vi "main.vi"() -> ()   [LabVIEW 2025]
uses:
  System.Windows.Forms
  TraceForwardLabviewAppTrace/Components/UIRefForHostInformation.ctl
  TraceForwardLabviewAppTrace/Components/MachineInterface/items/MachineState.ctl
  FormatData_ctl.ctl
  Mode_ctl.ctl
  TraceForwardLabviewAppTrace/Components/UIRefGlobal.vi
  TraceForwardLabviewAppTrace/Components/Config/items/GlobalConfigParam.vi
  <vilib>/NI/Modbus Library/API/Wrapper/Create Serial Master.vi
  <vilib>/NI/Modbus Library/API/Master/Modbus Master.lvclass
  <vilib>/Utility/config.llb/NI_LVConfig.lvlib
  TraceForwardLabviewAppTrace/Components/MachineInterface/MachineInterface.lvlib
  TraceForwardLabviewAppTrace/Components/HostInterface/HostInterface.lvlib
  TraceForwardLabviewAppTrace/Components/Logging/LogFunction.lvlib
  TraceForwardLabviewAppTrace/Components/Config/ConfigAppTraceFunction.lvlib
  <vilib>/NI/Modbus Library/API/Wrapper/API Main.lvlib
panel:
  out "Job ID":string
  out "QR code":string
  in  "Line":string
  out "标题":string="Nailer打钉功能测试"
  out "Assert Number":string
  out "Connection":bool
  out "HighAlarm":bool
  out "Energy(Wh)":dbl
  out "Power(W)":dbl
  out "Current(A)":dbl
  out "Error message":string
  out "register data":u16[](array[numeric])
  out "isOpen":bool
  out "FirstTime":bool
  out "Title":string
  out "Battery Low Voltage":bool
  out "Battery Voltage":dbl
  in  "Stop":bool
  in  "开始":bool caption="Start"
  out "PLC连接状态":bool caption="PLC Connection State"
  in  "型号":string(combo) caption="Model"
  in  "清零":bool caption="Reset"
  in  "Exit":bool
  in  "设置":bool caption="Setting"
  out "项目":string[][](table)
  out "波形图":waveform(dbl)(graph)
  out "进度条":u8(slide) scale=0.0..10.0
  in  "StatusStrip":refnum<k24>(container)
  # "v1.40"
  # "V"
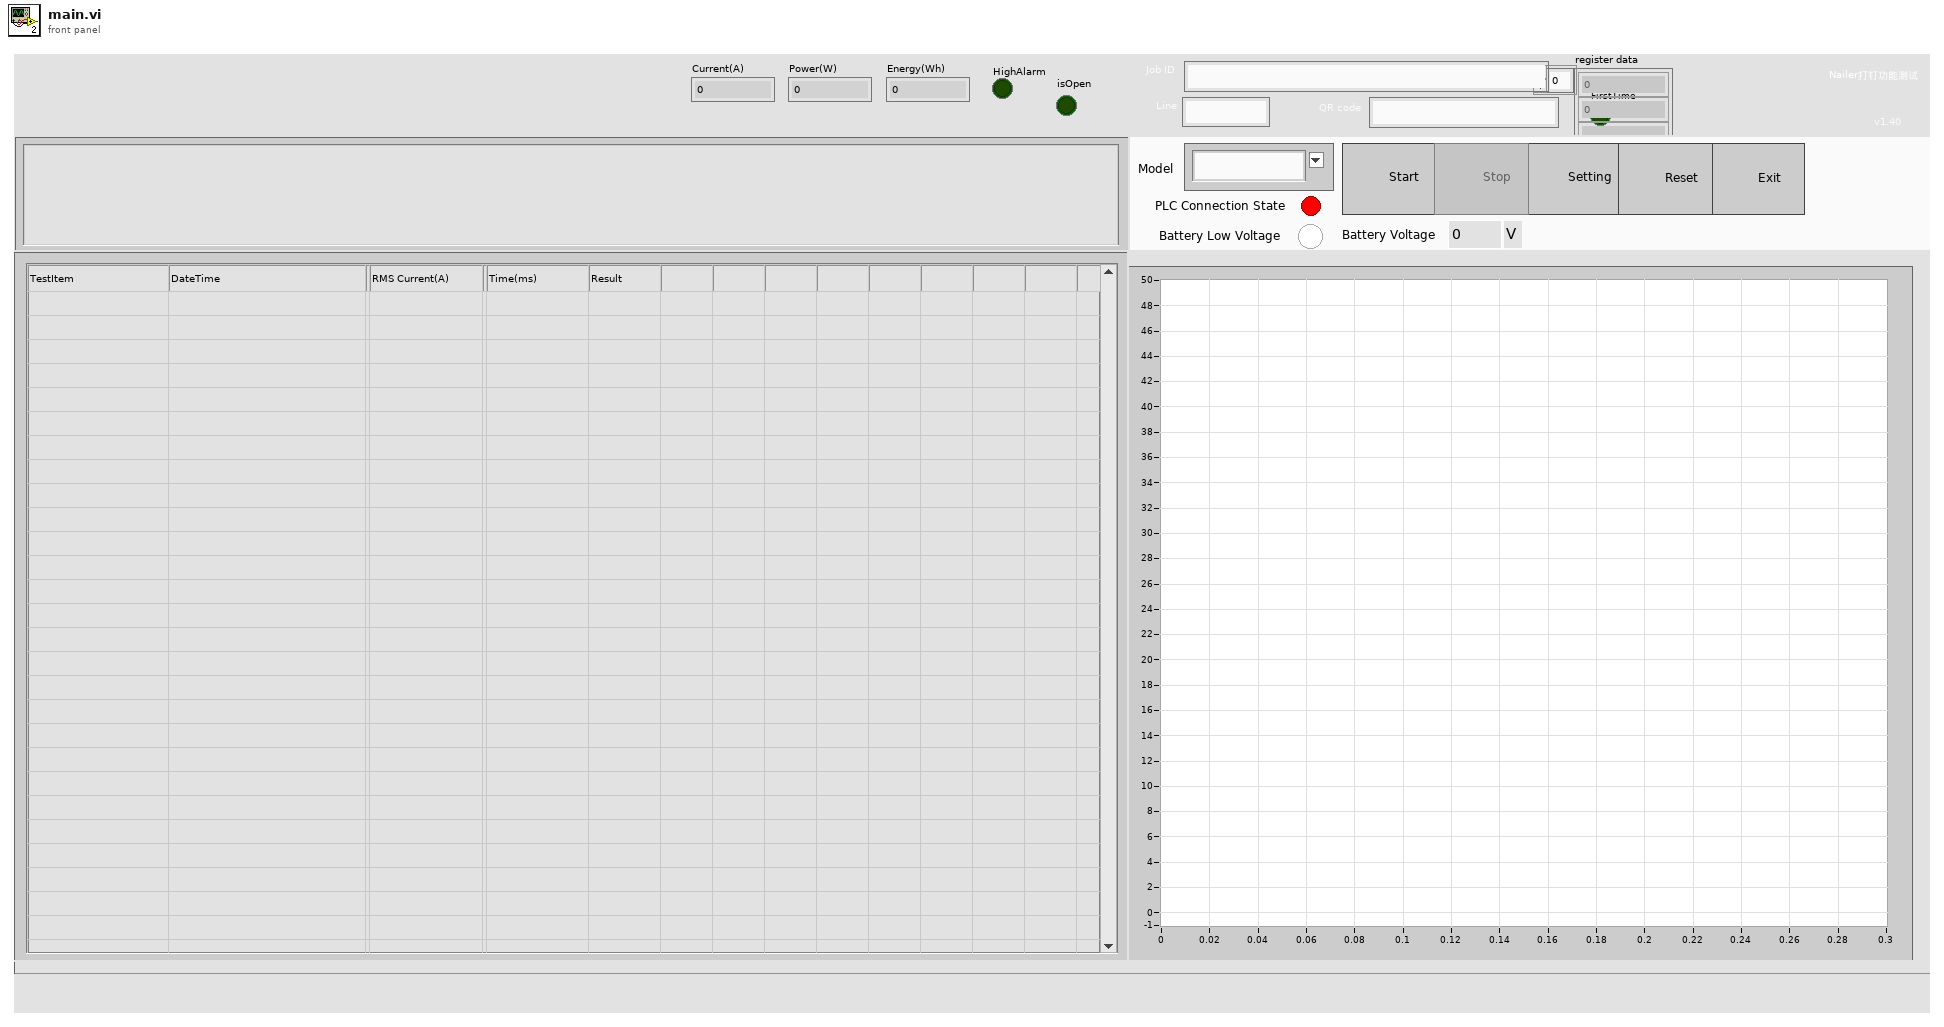
[diagram p1: front panel]
types:
  T1 = typedef "TraceForwardConnection.lvlib/MachineInterface.lvlib/UIRefForHostInformation.ctl" = cluster{"Lost Host Connection":refnum<vi>, "Error message":refnum<vi>, "Job ID":refnum<vi>, "QR":refnum<vi>, "Line id":refnum<vi>, "AssertNumber":refnum<vi>}
  T2 = cluster{"Text Color":u32, "Background Color":u32}
  T3 = enum32{"Invalid", "Standard", "Closed", "Hidden", "Minimized", "Maximized"}
  T4 = typedef "TraceForwardConnection.lvlib/MachineInterface.lvlib/MachineState.ctl" = enum16{"Reset", "Pre-start", "During test", "Data Ready", "OK_NG", "Stop", "WaitMC"}
  T5 = typedef "Mode_ctl.ctl" = enum16{"AddParam", "AddResult", "ReadData", "Clear"}
  T6 = typedef "FormatData_ctl.ctl" = cluster{"Max Current(A)":bool, "Avr Current(A)":bool, "Power":bool, "Time":bool, "Max Current(A) - UpLim":dbl, "Max Current(A) - MinLim":dbl, "Max Current(A) - RealValue":dbl, "Max Current(A) - Result":bool, "Avr Current(A) - UpLim":dbl, "Avr Current(A) - MinLim":dbl, "Avr Current(A) - RealValue":dbl, "Avr Current(A) - Result":bool, "Power- UpLim":dbl, "Power - MinLim":dbl, "Power- RealValue":dbl, "Power - Result":bool, "Time - UpLim":dbl, "Time - MinLim":dbl, "Time-RealValue":dbl, "Time - Result":bool}
  T7 = typedef "NI_LVConfig.lvlib/Config Data RefNum.ctl" = refnum<k1>
  T8 = cluster{"最大电流":bool, "平均电流":bool, "能量":bool, "打钉时间":bool, "单发打钉次数":u32, "连发打钉次数":u32, "触发值":dbl, "平均电流上限":dbl, "平均电流下限":dbl, "最大电流上限":dbl, "最大电流下限":dbl, "能量上限":dbl, "能量下限":dbl, "时间上限":dbl, "时间下限":dbl, "停止值":dbl, "倍数":dbl, "最大补偿":dbl, "平均补偿":dbl, "能量补偿":dbl, "时间补偿":dbl, "检查数":u32, "CurrentType":enum16{"RMS均方根值", "AVG平均值"}}
  T9 = cluster{"Name":string, "Type":string, "DefVal":string}[]
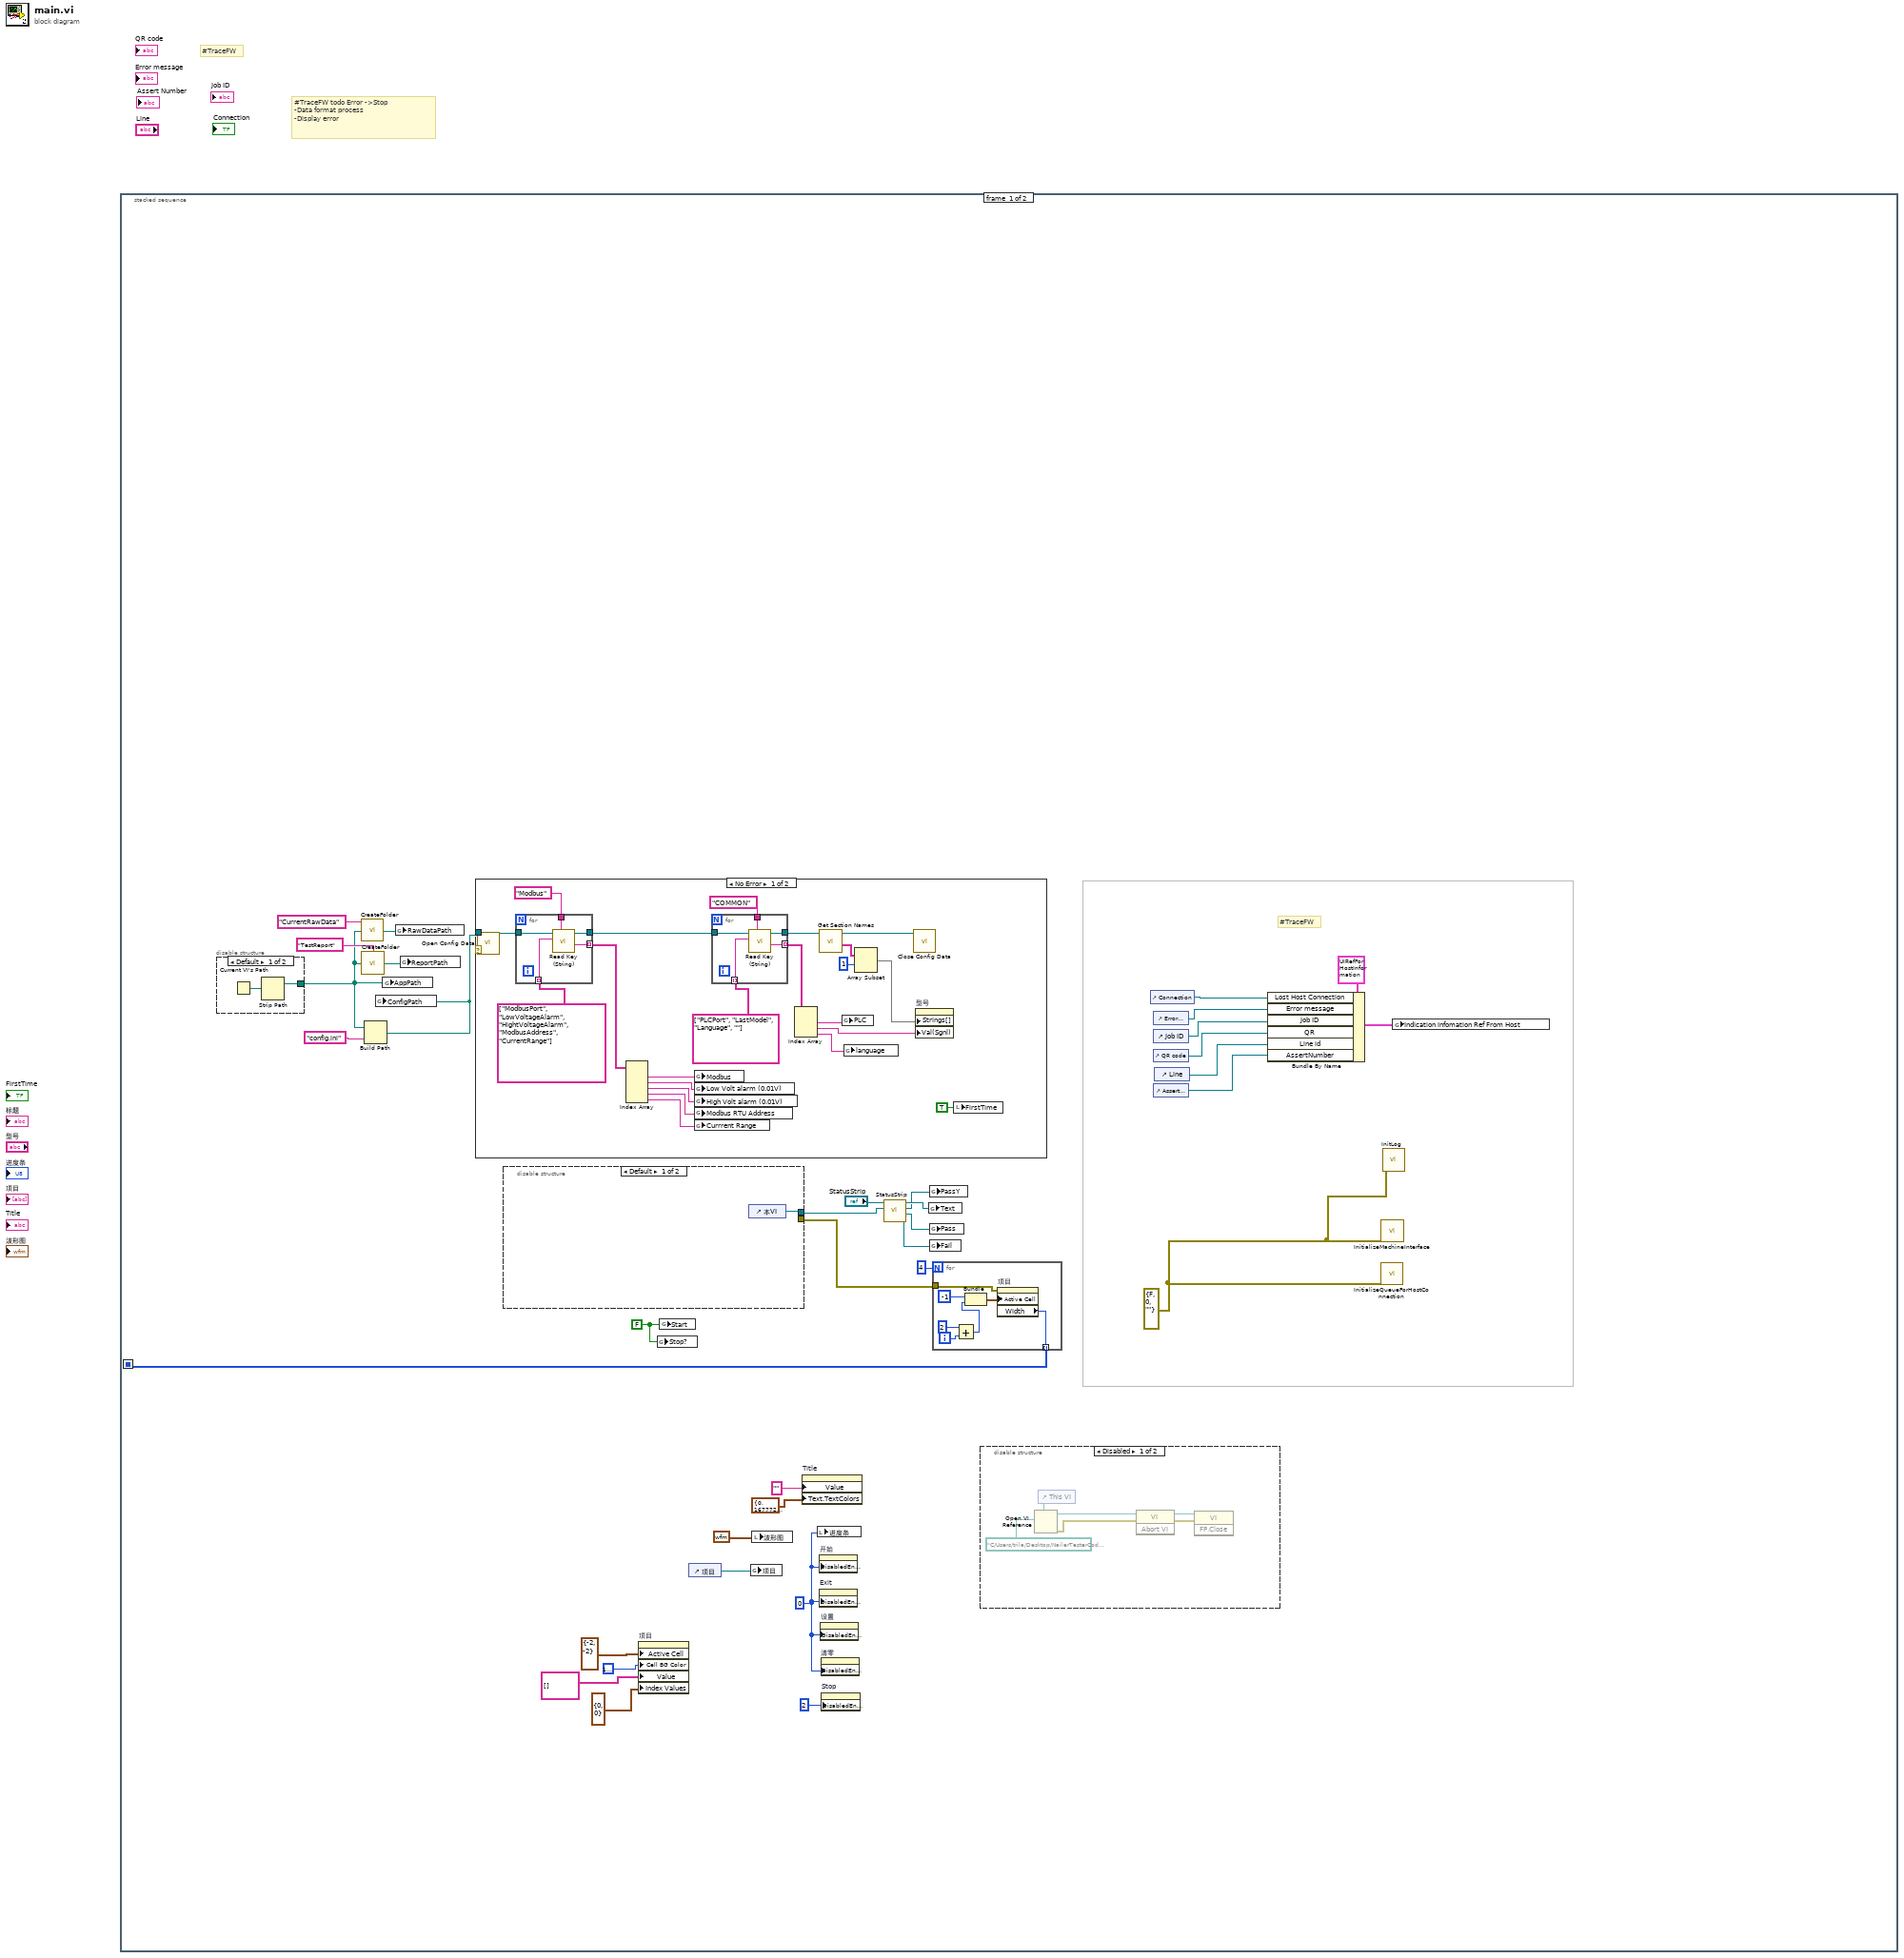
[diagram p0: block diagram]
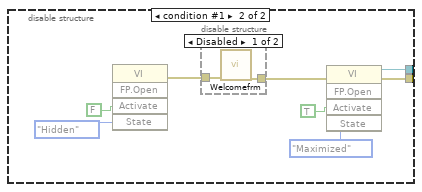
[diagram p3: hidden frame]
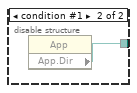
[diagram p5: hidden frame]
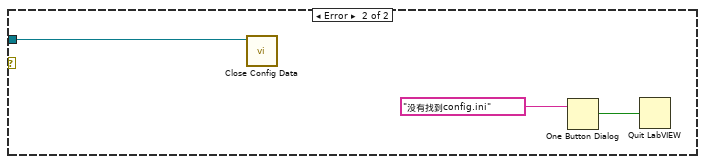
[diagram p6: hidden frame]
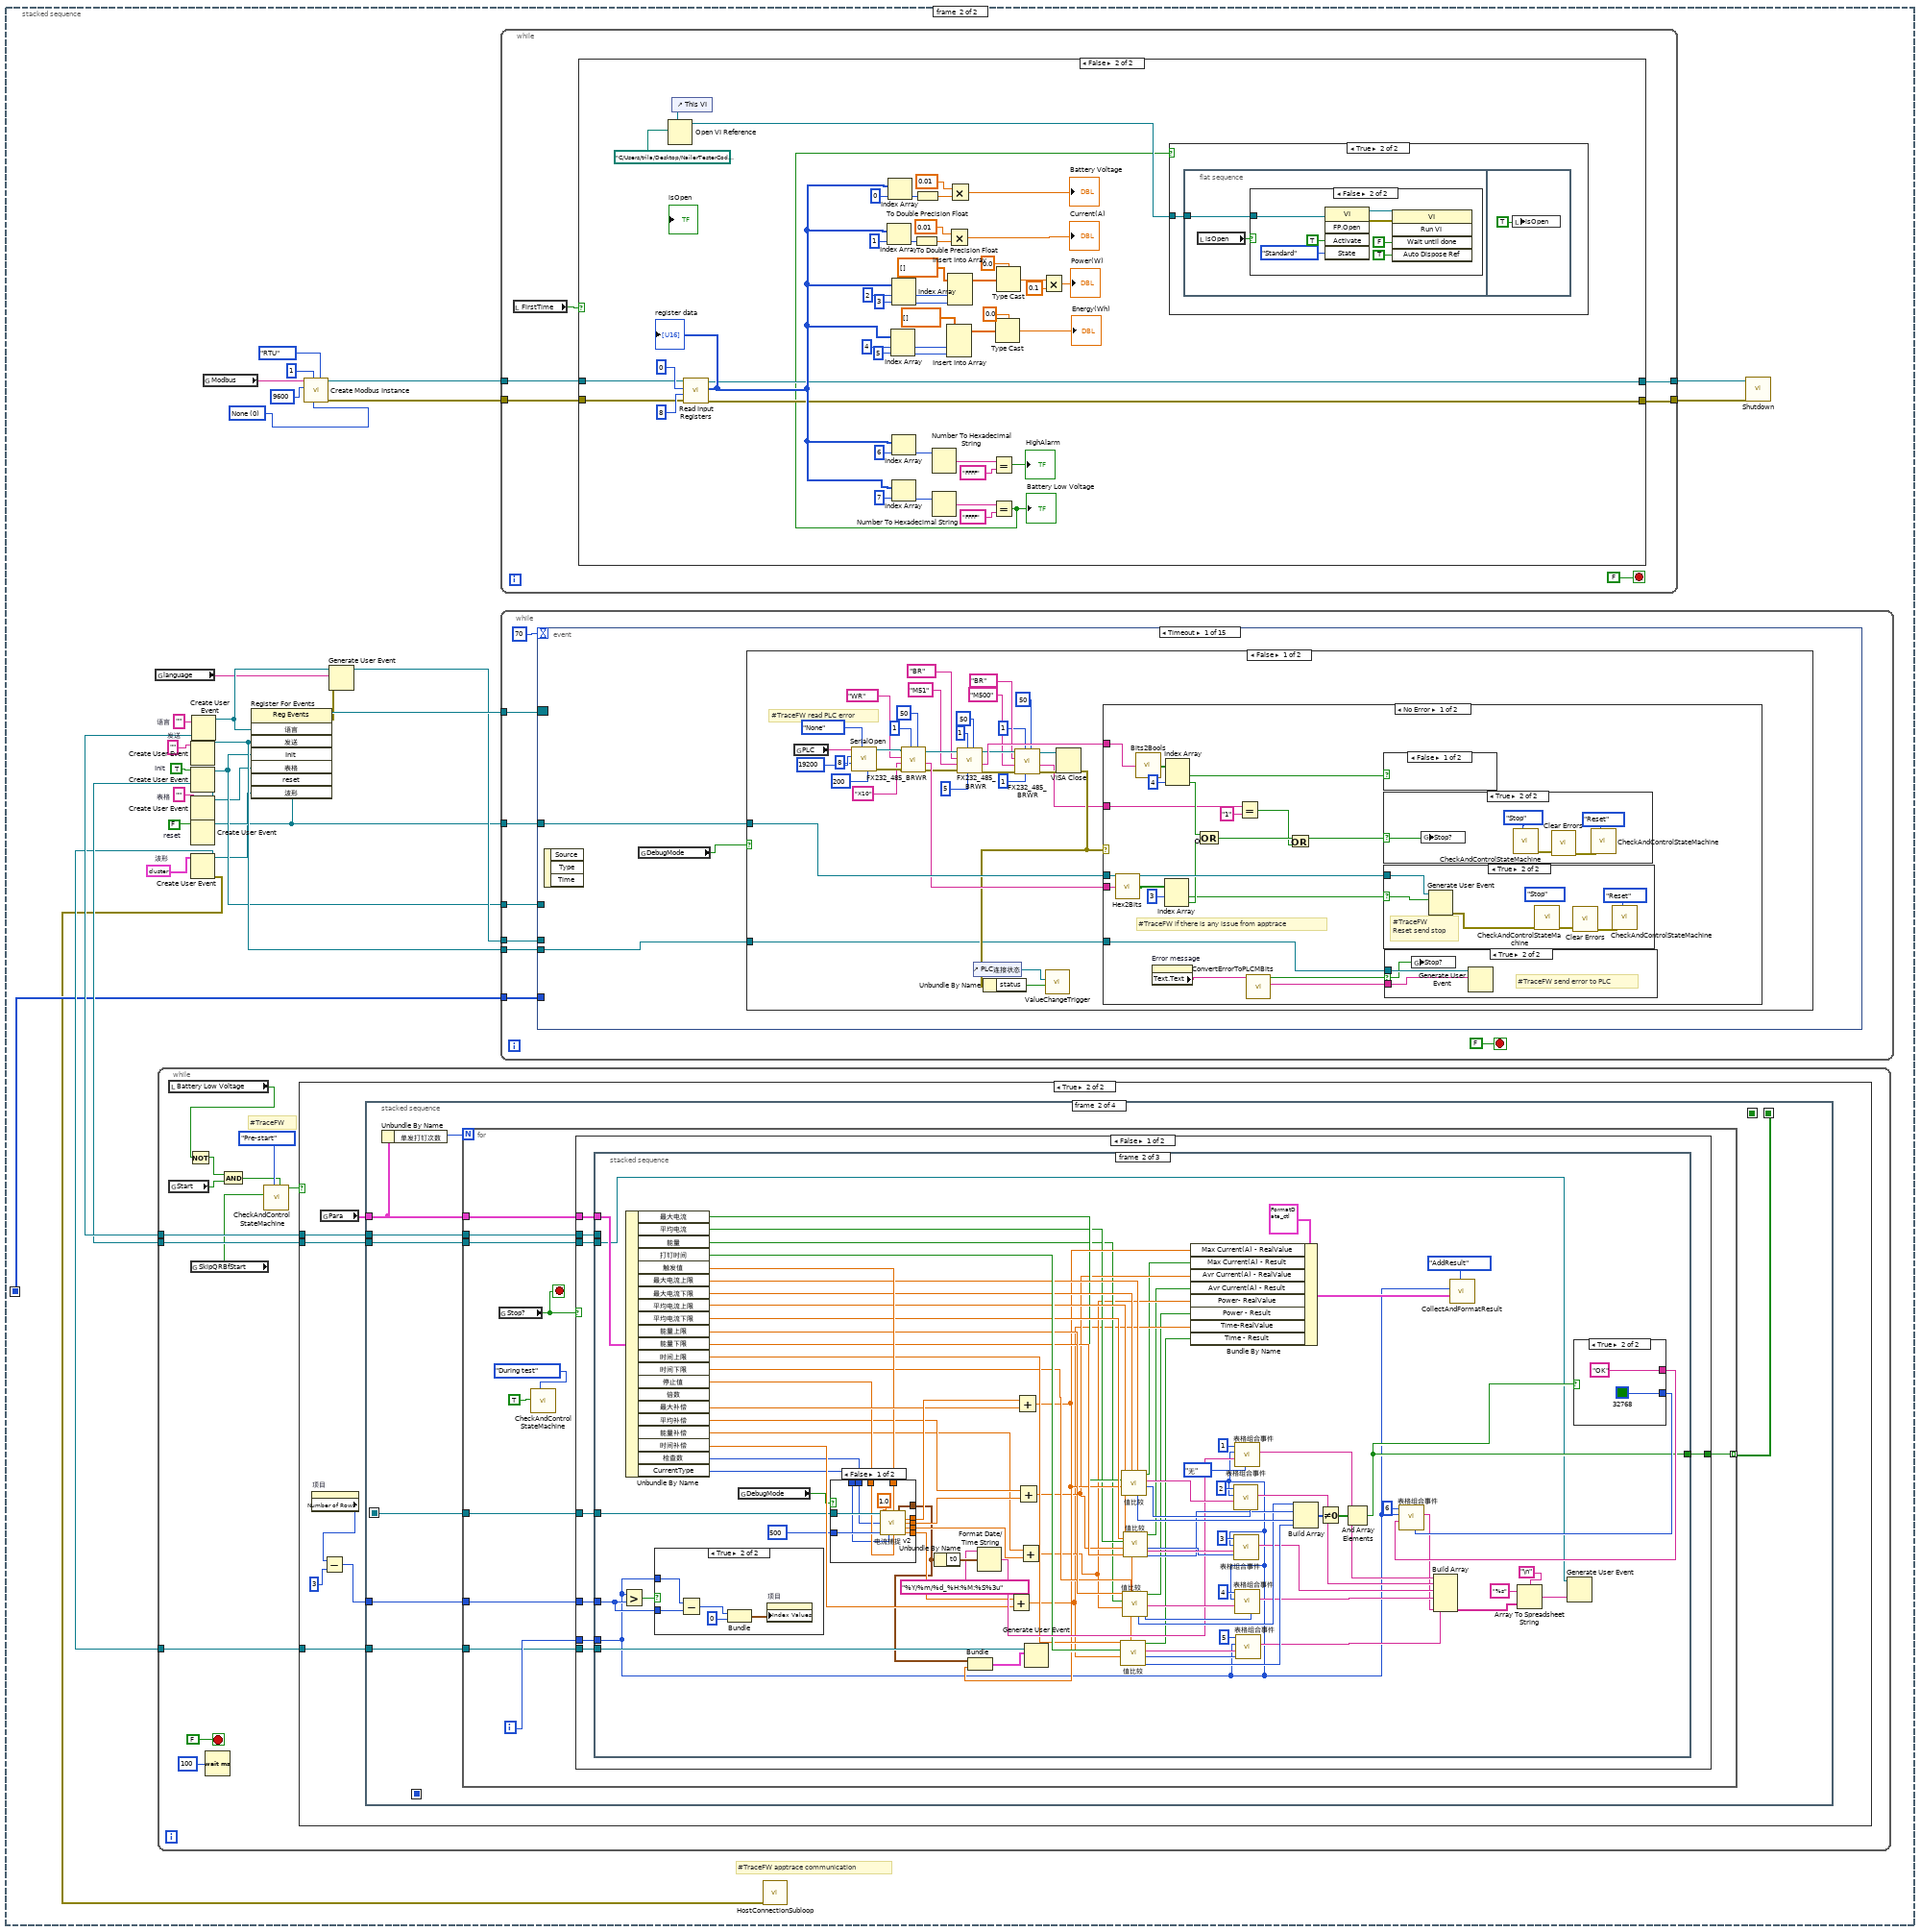
[diagram p7: hidden frame]
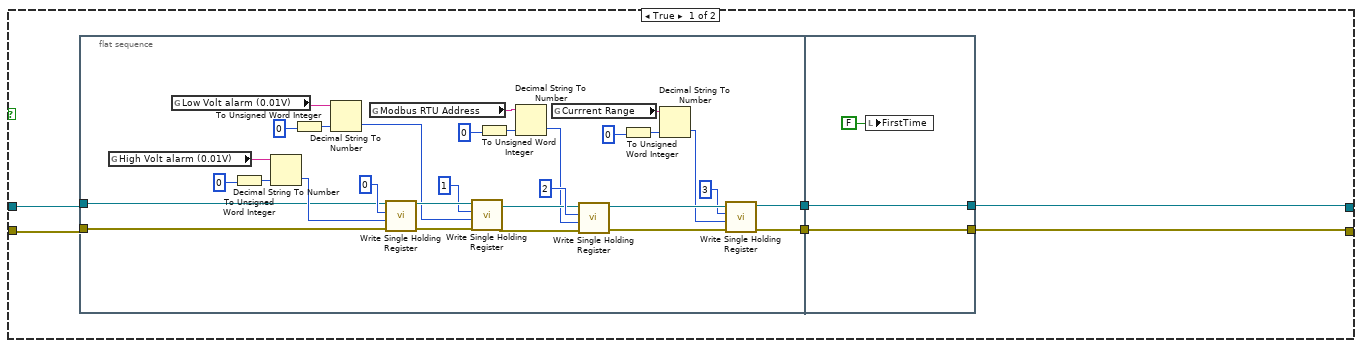
[diagram p8: hidden frame]
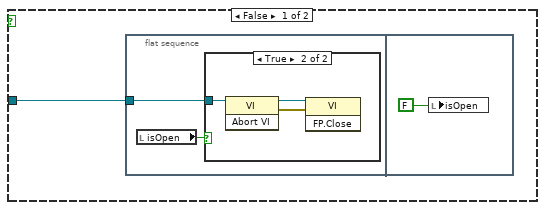
[diagram p9: hidden frame]
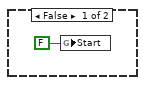
[diagram p12: hidden frame]
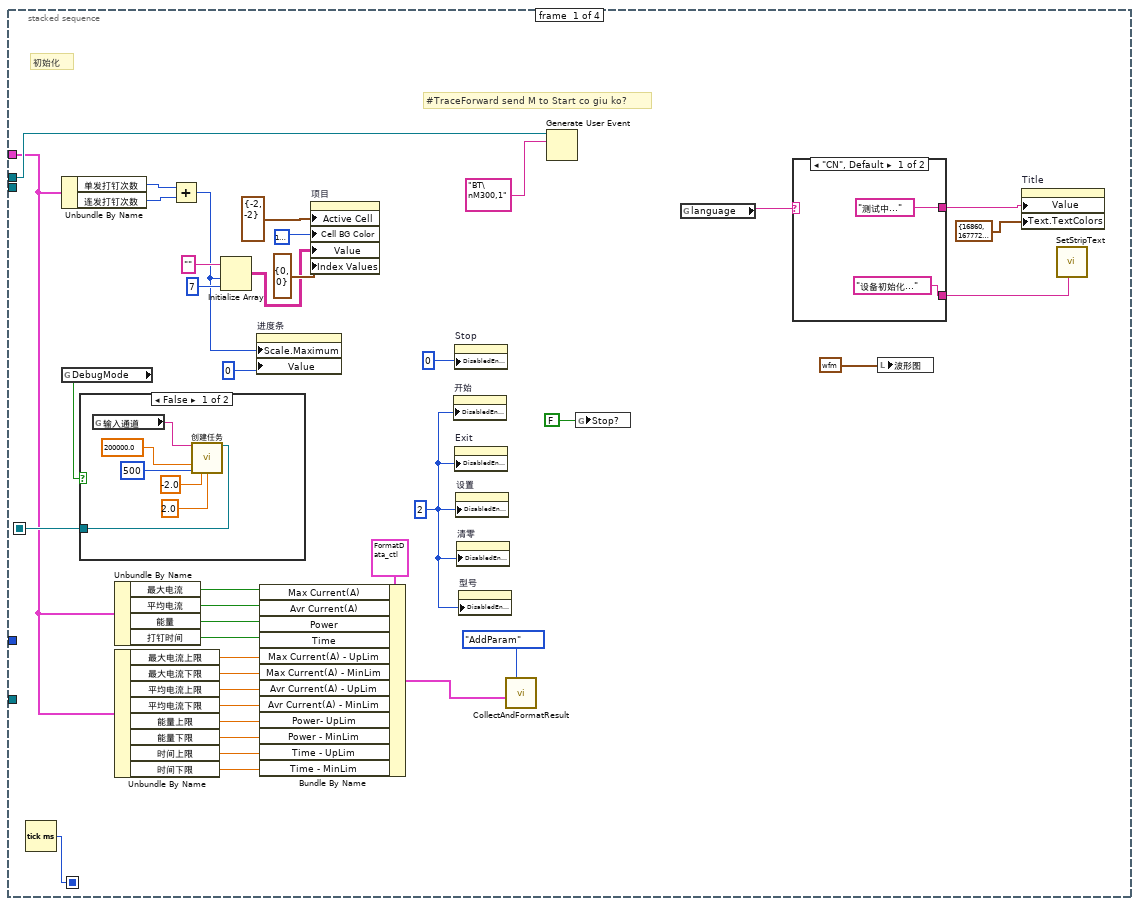
[diagram p13: hidden frame]
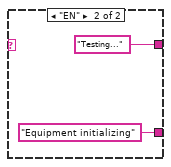
[diagram p15: hidden frame]
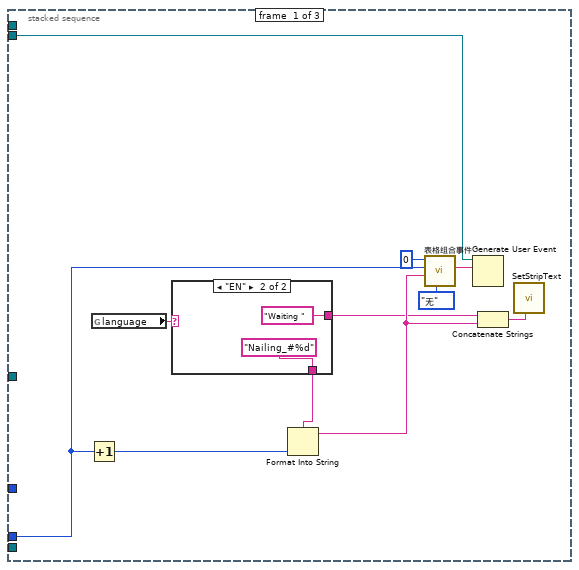
[diagram p16: hidden frame]
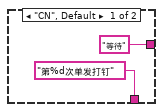
[diagram p17: hidden frame]
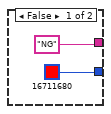
[diagram p20: hidden frame]
diagram:
  # "#TraceFW todo Error ->Stop\n-Data format process\n-Display error"
  # "#TraceFW"
  n1 = stacked-sequence {
    seq-local: [w15 _] -> [_ w113]
    frame #0 {
      w5 = errorcluster {"status"=FALSE, "code"=0, "source"=""} ("error in (no error)")
      w16 = 0
      w18 = FALSE ("InMain")
      # "#TraceFW"
      n2 = disable-structure shown="Default" {
        disable-tunnel: [w64 w66] -> w3
        frame condition #0 (active) {
          n3 = Current VI's Path() -> (path=w65:path)
          n4 = Strip Path(path=w65) -> (stripped path=w64:path)  [unwired: 1 out]
        }
        frame condition #1 {
          n5 = property class="App"() -> ("App.Dir"=w66:path)  [unwired: 2 in, 2 out]
        }
      }
      n6 = call "CreateFolder.vi"("folder name"="CurrentRawData", "Path in"=w3) -> ("path out"=w1:path)  [unwired: 2 in]
      n7 = call "CreateFolder.vi"("folder name"="TestReport" ("名称或相对路径"), "Path in"=w3) -> ("path out"=w22:path)  [unwired: 2 in]
      n8 = Build Path(base path=w3, name or relative path="config.ini" ("名称或相对路径")) -> (appended path=w20:path)
      n9 = global write "global.vi" "ConfigPath"(w20) -> ()
      n10 = global write "global.vi" "AppPath"(w3) -> ()
      n11 = global write "global.vi" "RawDataPath"(w1) -> ()
      n12 = global write "global.vi" "ReportPath"(w22) -> ()
      n13 = call <vilib>:"Open Config Data.vi"("configuration file path"=w20) -> ("error out"=w34:errorcluster, "refnum"=w33:T7)  [unwired: 8 in, 1 out]
      n14 = case shown="No Error" w34 {
        tunnel: w33 -> [w77 w99]
        frame No Error {
          n15 = for {
            tunnel: w77 -> [w93]
            tunnel: "Modbus" ("section") -> [w92]
            tunnel: string[] ["ModbusPort", "LowVoltageAlarm", "HightVoltageAlarm", "ModbusAddress", "CurrentRange"] -> [w91] mode=indexing
            tunnel: [w90] -> w73
            tunnel: [w89] -> w74 mode=indexing
            n16 = call <vilib>:"Read Key (String).vi"("section"=w92, "key"=w91, "refnum"=w93) -> ("value"=w89:string, "refnum out"=w90:T7)  [unwired: 5 in, 2 out]
          }
          n17 = Index Array(array=w74) -> (element #1=w72:string, element #2=w71:string, element #3=w70:string, element #4=w69:string, element #5=w68:string)  [unwired: 5 in]
          n18 = global write "global.vi" "Modbus"(w72) -> ()
          n19 = global write "global.vi" "Low Volt alarm (0.01V)"(w71) -> ()
          n20 = global write "global.vi" "High Volt alarm (0.01V)"(w70) -> ()
          n21 = global write "global.vi" "Modbus RTU Address"(w69) -> ()
          n22 = global write "global.vi" "Currrent Range"(w68) -> ()
          n23 = for {
            tunnel: w73 -> [w98]
            tunnel: "COMMON" ("section") -> [w97]
            tunnel: string[] ["PLCPort", "LastModel", "Language", ""] -> [w96] mode=indexing
            tunnel: [w95] -> w83
            tunnel: [w94] -> w87 mode=indexing
            n24 = call <vilib>:"Read Key (String).vi"("section"=w97, "key"=w96, "refnum"=w98) -> ("value"=w94:string, "refnum out"=w95:T7)  [unwired: 5 in, 2 out]
          }
          n25 = Index Array(array=w87) -> (element #1=w85:string, element #2=w78:string, element #3=w84:string)  [unwired: 3 in]
          n26 = call <vilib>:"Get Section Names.vi"("refnum"=w83) -> ("section names"=w82:string[], "refnum out"=w79:T7)  [unwired: 8 in, 1 out]
          n27 = global write "global.vi" "PLC"(w85) -> ()
          n28 = global write "global.vi" "language"(w84) -> ()
          n29 = Array Subset(array=w82, index=1 ("索引")) -> (w80:string[])  [unwired: 1 in]
          n30 = call <vilib>:"Close Config Data.vi"("refnum"=w79) -> ()  [unwired: 9 in, 2 out]
          n31 = property on="型号" class="CmbBox"("Strings[]"=w80, "Val(Sgnl)"=w78) -> ()  [unwired: 2 in, 2 out]
          n32 = local write "FirstTime"(TRUE ("FirstTime")) -> ()
        }
        frame Error {
          n33 = call <vilib>:"Close Config Data.vi"("refnum"=w99) -> ()  [unwired: 9 in, 2 out]
          n34 = One Button Dialog(message="没有找到config.ini" ("消息")) -> (true=w100:bool)  [unwired: 1 in]
          n35 = Quit LabVIEW(quit? (T)=w100) -> ()
        }
      }
      n36 = disable-structure shown="Default" {
        disable-tunnel: [w45 w48] -> w31
        disable-tunnel: [_ w47] -> w14
        frame condition #0 (active) {
          n37 = control-ref of="本VI"() -> (w45:refnum<vi>)
        }
        frame condition #1 {
          n38 = invoke class="VI" method="FP.Open"("Activate"=FALSE ("激活？"), "State"=T3."Hidden" ("状态")) -> (error out=w49:errorcluster)  [unwired: 3 in, 4 out]
          n39 = disable-structure shown="Disabled" {
            disable-tunnel: [w55 w56] -> w52
            disable-tunnel: w49 -> [w54 w56]
            frame Disabled {
              n40 = call "Welcomefrm.vi"("error in"=w54) -> ("error out"=w55:errorcluster)  [unwired: 10 in]
            }
            frame Enabled {
            }
          }
          n41 = invoke class="VI" method="FP.Open"(error in=w52, "Activate"=TRUE ("激活？"), "State"=T3."Maximized" ("状态")) -> (reference out=w48:refnum<vi>, error out=w47:errorcluster)  [unwired: 2 in, 3 out]
        }
      }
      n42 = property on="项目" class="Tbl (strict)"("Active Cell"=cluster{"Row":i32, "Column":i32} {"Row"=-2, "Column"=-2} ("活动单元格:活动单元格"), "Cell BG Color"=u32 16777225, "Value"=string[][] [] ("项目 2"), "Index Values"=cluster{"Row":u32, "Column":u32} {"Row"=0, "Column"=0} ("索引值")) -> ()  [unwired: 2 in, 2 out]
      n43 = global write "global.vi" "Stop?"(w18) -> ()
      n44 = global write "global.vi" "Start"(w18) -> ()
      n45 = control-ref of="项目"() -> (w27:refnum<vi>)
      n46 = global write "global.vi" "项目"(w27) -> ()
      n47 = local write "波形图"(waveform(dbl) {"t0"=timestamp(0 s since 1904-01-01), "dt"=1.0, "Y"=[]} ("Waveform")) -> ()
      n48 = property on="Title" class="Str"("Value"="" ("Title"), "Text.TextColors"=T2 {"Text Color"=0, "Background Color"=16777225} ("文本.文本颜色")) -> ()  [unwired: 2 in, 2 out]
      n49 = local write "进度条"(w16) -> ()
      n50 = property on="开始" class="Bool"("DisabledEnum"=w16) -> ()  [unwired: 2 in, 2 out]
      n51 = property on="Exit" class="Bool"("DisabledEnum"=w16) -> ()  [unwired: 2 in, 2 out]
      n52 = property on="设置" class="Bool"("DisabledEnum"=w16) -> ()  [unwired: 2 in, 2 out]
      n53 = property on="清零" class="Bool"("DisabledEnum"=w16) -> ()  [unwired: 2 in, 2 out]
      n54 = property on="Stop" class="Bool"("DisabledEnum"=2) -> ()  [unwired: 2 in, 2 out]
      n55 = call "StatusStrip.vi"("VI引用"=w31, "StatusStrip"="StatusStrip") -> ("Fail"=w38:refnum<k24>, "Pass"=w37:refnum<k24>, "PassY"=w32:refnum<k24>, "Text"=w36:refnum<k24>)  [unwired: 6 in]
      n56 = global write "global.vi" "Text"(w36) -> ()
      n57 = global write "global.vi" "PassY"(w32) -> ()
      n58 = global write "global.vi" "Pass"(w37) -> ()
      n59 = global write "global.vi" "Fail"(w38) -> ()
      n60 = for {
        N: 4 -> [_]
        tunnel: [w61] -> w15 mode=indexing
        tunnel: w14 -> [w60]
        i -> [w59]
        n61 = Add(x=2, y=w59) -> (x+y=w57:i32)
        n62 = Bundle(-1, w57) -> (w62:cluster{i32, i32})  [unwired: 1 in]
        n63 = property on="项目" class="Tbl (strict)"(error in=w60, "Active Cell"=w62) -> ("Width"=w61:u32)  [unwired: 1 in, 2 out]
      }
      n64 = disable-structure shown="Disabled" {
        frame Disabled {
          n65 = control-ref of="This VI"() -> (w44:refnum<vi>)
          n66 = Open VI Reference(type specifier VI Refnum (for type only)=w44, vi path=path "C:/Users/trila/Desktop/NailerTesterCode_ApplyTrace/NailerTesterCode/Alarm_Battery.vi") -> (vi reference=w40:refnum<vi>, error out=w39:errorcluster)  [unwired: 4 in]
          n67 = invoke class="VI" method="Abort VI"(reference=w40, error in=w39) -> (reference out=w42:refnum<vi>, error out=w41:errorcluster)  [unwired: 1 in, 1 out]
          n68 = invoke class="VI" method="FP.Close"(reference=w42, error in=w41) -> ()  [unwired: 1 in, 3 out]
        }
        frame Enabled {
        }
      }
      n69 = control-ref of="Connection"() -> (w10:refnum<vi>)
      n70 = control-ref of="Error message"() -> (w9:refnum<vi>)
      n71 = control-ref of="Job ID"() -> (w8:refnum<vi>)
      n72 = control-ref of="QR code"() -> (w4:refnum<vi>)
      n73 = control-ref of="Assert Number"() -> (w6:refnum<vi>)
      n74 = control-ref of="Line"() -> (w7:refnum<vi>)
      n75 = Bundle By Name(cluster=T1 {"Lost Host Connection"=refnum, "Error message"=refnum, "Job ID"=refnum, "QR"=refnum, "Line id"=refnum, "AssertNumber"=refnum} ("UIRefForHostInfomation"), "Lost Host Connection"=w10, "Error message"=w9, "Job ID"=w8, "QR"=w4, "Line id"=w7, "AssertNumber"=w6) -> (w11:T1)
      n76 = call "InitializeQueueForHostConnection.vi"("error in (no error)"=w5) -> ()  [unwired: 9 in, 2 out]
      n77 = call "InitializeMachineInterface.vi"("error in (no error)"=w5) -> ()  [unwired: 10 in, 1 out]
      n78 = call "InitLog.vi"("error in (no error)"=w5) -> ()  [unwired: 10 in, 1 out]
      n79 = global write "UIRefGlobal.vi" "Indication Infomation Ref From Host"(w11) -> ()
    }
    frame #1 {
      w108 = u16 0 items=["None", "Odd", "Even", "Mark", "Space"] ("parity (even)")
      w112 = ""  # 发送
      w114 = cluster{"Waveform":waveform(dbl), "最大电流":dbl} {"Waveform"={"t0"=timestamp(0 s since 1904-01-01), "dt"=1.0, "Y"=[]}, "最大电流"=0.0}  # 波形
      w117 = FALSE  # reset
      w119 = ""  # 表格
      w126 = ""  # 语言
      w127 = TRUE  # Init
      # "#TraceFW apptrace communication"
      n80 = global read "global.vi" "language"() -> (w122:string)
      n81 = Create User Event(user event datatype=w112) -> (user event=w121:refnum<user-event>)  [unwired: 1 in, 1 out]
      n82 = Create User Event(user event datatype=w127) -> (user event=w120:refnum<user-event>)  [unwired: 1 in, 1 out]
      n83 = Create User Event(user event datatype=w119) -> (user event=w118:refnum<user-event>)  [unwired: 1 in, 1 out]
      n84 = Create User Event(user event datatype=w117) -> (user event=w116:refnum<user-event>)  [unwired: 1 in, 1 out]
      n85 = Create User Event(user event datatype=w114) -> (user event=w115:refnum<user-event>, error out=w111:errorcluster)  [unwired: 1 in]
      n86 = while {
        tunnel: w121 -> [w249]
        tunnel: w118 -> [w248]
        tunnel: w115 -> [w247]
        stop <- FALSE stop-if-true
        # "#TraceFW"
        n87 = local read "Battery Low Voltage"() -> (w243:bool)
        n88 = global read "global.vi" "Start"() -> (w241:bool)
        n89 = Not(x=w243) -> (.not. x?=w242:bool)
        n90 = global read "GlobalConfigParam.vi" "SkipQRBfStart"() -> (w244:bool)
        n91 = Wait (ms)(milliseconds to wait=u32 100 ("等待时间（毫秒）")) -> ()  [unwired: 1 out]
        n92 = And(x=w242, y=w241) -> (x .and. y?=w240:bool)
        n93 = call "CheckAndControlStateMachine.vi"("Send?"=w240, "Mode"=MachineState."Pre-start", "SkipQRcheck"=w244) -> ("Change State OK"=w245:bool)  [unwired: 5 in, 3 out]
        n94 = case shown="True" w245 {
          tunnel: w249 -> [_ w258]
          tunnel: w248 -> [_ w254]
          tunnel: w247 -> [_ w253]
          frame False {
            n95 = global write "global.vi" "Start"(FALSE ("Start")) -> ()
          }
          frame True {
            n96 = property on="项目" class="Tbl (strict)"() -> ("Number of Rows"=w256:u32)  [unwired: 2 in, 2 out]
            n97 = global read "global.vi" "Para"() -> (w259:T8)
            n98 = Subtract(x=w256, y=u32 3) -> (x-y=w257:u32)
            n99 = stacked-sequence {
              seq-local: [w293 _ _ _] -> [_ _ _ w695]
              seq-local: [_ w315 _ _] -> [_ _ _ w671]
              seq-local: [_ _ w494 _] -> [_ _ _ w669]
              seq-local: [w283 _ _ _] -> [_ w310 w485 w665]
              tunnel: w259 -> [w270 w316 w495 _]
              tunnel: w258 -> [w277 w313 w488 w667]
              tunnel: w257 -> [_ w312 w487 _]
              tunnel: w254 -> [_ w311 w486 _]
              tunnel: w253 -> [_ w309 w484 _]
              frame #0 {
                w282 = u8 2
                # "#TraceForward send M to Start co giu ko?"
                # "初始化"
                n100 = Tick Count (ms)() -> (millisecond timer value=w293:u32)
                n101 = Unbundle By Name(w270) -> ("单发打钉次数"=w297:u32, "连发打钉次数"=w296:u32)
                n102 = global read "GlobalConfigParam.vi" "DebugMode"() -> (w276:bool)
                n103 = case shown="False" w276 {
                  tunnel: [w299 _] -> w283
                  frame False {
                    n104 = global read "global.vi" "输入通道"() -> (w300:tag)
                    n105 = call "创建任务.vi"("输入通道"=w300, "速率"=200000.0, "采样数"=500, "最小输入值"=-2.0, "最大输入值"=2.0) -> ("task out"=w299:refnum<k21>)  [unwired: 8 in, 2 out]
                  }
                  frame True {
                  }
                }
                n106 = Unbundle By Name(w270) -> ("最大电流"=w274:bool, "平均电流"=w273:bool, "能量"=w272:bool, "打钉时间"=w271:bool)
                n107 = Unbundle By Name(w270) -> ("最大电流上限"=w269:dbl, "最大电流下限"=w268:dbl, "平均电流上限"=w267:dbl, "平均电流下限"=w266:dbl, "能量上限"=w265:dbl, "能量下限"=w264:dbl, "时间上限"=w263:dbl, "时间下限"=w262:dbl)
                n108 = Add(x=w297, y=w296) -> (x+y=w291:u32)
                n109 = Initialize Array("", w291, 7 ("维数大小")) -> (w285:string[][])
                n110 = property on="进度条" class="Slide (strict)"("Scale.Maximum"=w291, "Value"=u8 0 ("进度条")) -> ()  [unwired: 2 in, 2 out]
                n111 = Bundle By Name(cluster=T6 {"Max Current(A)"=FALSE, "Avr Current(A)"=FALSE, "Power"=FALSE, "Time"=FALSE, "Max Current(A) - UpLim"=0.0, "Max Current(A) - MinLim"=0.0, "Max Current(A) - RealValue"=0.0, "Max Current(A) - Result"=FALSE, "Avr Current(A) - UpLim"=0.0, "Avr Current(A) - MinLim"=0.0, "Avr Current(A) - RealValue"=0.0, "Avr Current(A) - Result"=FALSE, "Power- UpLim"=0.0, "Power - MinLim"=0.0, "Power- RealValue"=0.0, "Power - Result"=FALSE, "Time - UpLim"=0.0, "Time - MinLim"=0.0, "Time-RealValue"=0.0, "Time - Result"=FALSE}, "Max Current(A)"=w274, "Avr Current(A)"=w273, "Power"=w272, "Time"=w271, "Max Current(A) - UpLim"=w269, "Max Current(A) - MinLim"=w268, "Avr Current(A) - UpLim"=w267, "Avr Current(A) - MinLim"=w266, "Power- UpLim"=w265, "Power - MinLim"=w264, "Time - UpLim"=w263, "Time - MinLim"=w262) -> (w260:T6)
                n112 = property on="项目" class="Tbl (strict)"("Active Cell"=cluster{"Row":i32, "Column":i32} {"Row"=-2, "Column"=-2} ("活动单元格:活动单元格"), "Cell BG Color"=u32 16777225, "Value"=w285, "Index Values"=cluster{"Row":u32, "Column":u32} {"Row"=0, "Column"=0} ("索引值")) -> ()  [unwired: 2 in, 2 out]
                n113 = property on="开始" class="Bool"("DisabledEnum"=w282) -> ()  [unwired: 2 in, 2 out]
                n114 = property on="Stop" class="Bool"("DisabledEnum"=0) -> ()  [unwired: 2 in, 2 out]
                n115 = property on="Exit" class="Bool"("DisabledEnum"=w282) -> ()  [unwired: 2 in, 2 out]
                n116 = property on="设置" class="Bool"("DisabledEnum"=w282) -> ()  [unwired: 2 in, 2 out]
                n117 = property on="清零" class="Bool"("DisabledEnum"=w282) -> ()  [unwired: 2 in, 2 out]
                n118 = property on="型号" class="CmbBox"("DisabledEnum"=w282) -> ()  [unwired: 2 in, 2 out]
                n119 = call "CollectAndFormatResult.vi"("Mode"=Mode_ctl."AddParam", "Param/Result"=w260) -> ()  [unwired: 9 in, 1 out]
                n120 = Generate User Event(user event=w277, event data cluster="BT\nM300,1") -> ()  [unwired: 2 in, 2 out]
                n121 = global write "global.vi" "Stop?"(FALSE ("Start")) -> ()
                n122 = global read "global.vi" "language"() -> (w281:string)
                n123 = case shown="\"CN\", Default" w281 {
                  tunnel: ["测试中..." ("Title") "Testing..." ("Title")] -> w280
                  tunnel: ["设备初始化..." ("Info") "Equipment initializing" ("Info")] -> w279
                  frame "CN", Default {
                  }
                  frame "EN" {
                  }
                }
                n124 = local write "波形图"(waveform(dbl) {"t0"=timestamp(0 s since 1904-01-01), "dt"=1.0, "Y"=[]} ("Waveform")) -> ()
                n125 = property on="Title" class="Str"("Value"=w280, "Text.TextColors"=T2 {"Text Color"=16860, "Background Color"=16777225} ("文本.文本颜色")) -> ()  [unwired: 2 in, 2 out]
                n126 = call "SetStripText.vi"("Info"=w279) -> ()  [unwired: 8 in, 3 out]
              }
              frame #1 {
                n127 = Unbundle By Name(w316) -> ("单发打钉次数"=w314:u32)
                n128 = for {
                  N: w314 -> [_]
                  tunnel: w316 -> [w325]
                  tunnel: [w327] -> w315 mode=indexing
                  tunnel: w313 -> [w323]
                  tunnel: w312 -> [w322]
                  tunnel: w311 -> [w321]
                  tunnel: w310 -> [w320]
                  tunnel: w309 -> [w319]
                  i -> [w324]
                  stop <- w326 stop-if-true
                  n129 = global read "global.vi" "Stop?"() -> (w326:bool)
                  n130 = call "CheckAndControlStateMachine.vi"("Mode"=MachineState."During test", "SkipQRcheck"=TRUE) -> ()  [unwired: 6 in, 4 out]
                  n131 = case shown="False" w326 {
                    tunnel: w325 -> [w335 _]
                    tunnel: [w334 _] -> w327
                    tunnel: w324 -> [w333 _]
                    tunnel: w323 -> [w332 _]
                    tunnel: w322 -> [w331 _]
                    tunnel: w321 -> [w330 _]
                    tunnel: w320 -> [w329 _]
                    tunnel: w319 -> [w328 _]
                    frame False {
                      n132 = stacked-sequence {
                        tunnel: w333 -> [w342 w351 w456]
                        tunnel: w335 -> [_ w433 _]
                        tunnel: [_ w411 _] -> w334
                        tunnel: w332 -> [_ _ w477]
                        tunnel: w331 -> [_ w405 _]
                        tunnel: w330 -> [w340 w399 _]
                        tunnel: w329 -> [_ w388 _]
                        tunnel: w328 -> [_ w384 _]
                        frame #0 {
                          n133 = Increment(x=w342) -> (x+1=w341:i32)
                          n134 = global read "global.vi" "language"() -> (w338:string)
                          n135 = case shown="\"EN\"" w338 {
                            tunnel: ["第%d次单发打钉" ("格式字符串") "Nailing_#%d" ("格式字符串")] -> w337
                            tunnel: ["等待" "Waiting "] -> w336
                            frame "CN", Default {
                            }
                            frame "EN" {
                            }
                          }
                          n136 = Format Into String(format string=w337, w341) -> (resulting string=w345:string)  [unwired: 2 in, 1 out]
                          n137 = call "表格组合事件.vi"("类型"=enum16{"无", "单格", "整行", "整列"}."无", "字符串"=w345, "Row"=w342, "Col"=0) -> ("结果字符串"=w339:string)  [unwired: 7 in]
                          n138 = Generate User Event(user event=w340, event data cluster=w339) -> ()  [unwired: 2 in, 2 out]
                          n139 = Concatenate Strings(w336, w345) -> (w346:string)
                          n140 = call "SetStripText.vi"("Info"=w346) -> ()  [unwired: 8 in, 3 out]
                        }
                        frame #1 {
                          n141 = Greater?(x=w351, y=w405) -> (0:w406:bool)
                          n142 = Unbundle By Name(w433) -> ("最大电流"=w365:bool, "平均电流"=w363:bool, "能量"=w362:bool, "打钉时间"=w380:bool, "触发值"=w385:dbl, "最大电流上限"=w379:dbl, "最大电流下限"=w378:dbl, "平均电流上限"=w377:dbl, "平均电流下限"=w376:dbl, "能量上限"=w375:dbl, "能量下限"=w374:dbl, "时间上限"=w373:dbl, "时间下限"=w372:dbl, "停止值"=w386:dbl, "最大补偿"=w403:dbl, "平均补偿"=w371:dbl, "能量补偿"=w369:dbl, "时间补偿"=w401:dbl, "检查数"=w383:u32, "CurrentType"=w382:enum16{"RMS均方根值", "AVG平均值"})  [unwired: 1 out]
                          n143 = case shown="True" w406 {
                            tunnel: w351 -> [_ w448]
                            tunnel: w405 -> [_ w447]
                            frame False {
                            }
                            frame True {
                              n144 = Subtract(x=w448, y=w447) -> (x-y=w446:u32)
                              n145 = Bundle(w446, 0) -> (w449:cluster{u32, i32})  [unwired: 1 in]
                              n146 = property on="项目" class="Tbl (strict)"("Index Values"=w449) -> ()  [unwired: 2 in, 2 out]
                            }
                          }
                          n147 = global read "GlobalConfigParam.vi" "DebugMode"() -> (w381:bool)
                          n148 = case shown="False" w381 {
                            tunnel: [w445 _] -> w404
                            tunnel: [w444 _] -> w370
                            tunnel: [w443 _] -> w368
                            tunnel: [w442 _] -> w402
                            tunnel: w388 -> [w440 _]
                            tunnel: 500 ("采样数") -> [w439 _]
                            tunnel: w386 -> [w438 _]
                            tunnel: w385 -> [w437 _]
                            tunnel: [w436 _] -> w352
                            tunnel: w383 -> [w435 _]
                            tunnel: w382 -> [w434 _]
                            frame False {
                              n149 = call "电流捕捉 v2.vi"("task/channels in"=w440, "驱动值"=w437, "条件"=1.0, "停止次数"=w435, "采样数"=w439, "CurrentType"=w434, "停止值"=w438) -> ("输出波形"=w436:waveform(dbl), "最大电流"=w445:dbl, "电流值"=w444:dbl, "能量"=w443:dbl, "持续时间"=w442:dbl)  [unwired: 3 in, 1 out]
                            }
                            frame True {
                            }
                          }
                          n150 = Unbundle By Name(w352) -> ("t0"=w410:timestamp)
                          n151 = Format Date/Time String(time format string (%c)="%Y/%m/%d_%H:%M:%S%3u" ("时间格式字符串(%c)"), seconds (now)=w410) -> (date/time string=w408:string)  [unwired: 1 in]
                          n152 = Add(x=w402, y=w401) -> (x+y=w360:dbl)
                          n153 = Add(x=w404, y=w403) -> (x+y=w366:dbl)
                          n154 = Bundle("输出波形"=w352, w366) -> (w353:cluster{"输出波形":waveform(dbl), dbl})  [unwired: 1 in]
                          n155 = Add(x=w371, y=w370) -> (x+y=w364:dbl)
                          n156 = Add(x=w369, y=w368) -> (x+y=w361:dbl)
                          n157 = Generate User Event(user event=w384, event data cluster=w353) -> ()  [unwired: 2 in, 2 out]
                          n158 = call "值比较.vi"("上限"=w373, "下限"=w372, "x"=w360, "s"=w380) -> ("颜色盒"=w425:u32, "值"=w426:string, "Pass(T)/Fail(F)"=w359:bool, "结果"=w416:enum16{"Failed", "Passed", "Disabled"})  [unwired: 4 in]
                          n159 = call "值比较.vi"("上限"=w379, "下限"=w378, "x"=w366, "s"=w365) -> ("颜色盒"=w427:u32, "值"=w428:string, "Pass(T)/Fail(F)"=w358:bool, "结果"=w419:enum16{"Failed", "Passed", "Disabled"})  [unwired: 4 in]
                          n160 = call "值比较.vi"("上限"=w375, "下限"=w374, "x"=w361, "s"=w362) -> ("颜色盒"=w423:u32, "值"=w424:string, "Pass(T)/Fail(F)"=w356:bool, "结果"=w417:enum16{"Failed", "Passed", "Disabled"})  [unwired: 4 in]
                          n161 = call "值比较.vi"("上限"=w377, "下限"=w376, "x"=w364, "s"=w363) -> ("颜色盒"=w421:u32, "值"=w422:string, "Pass(T)/Fail(F)"=w357:bool, "结果"=w418:enum16{"Failed", "Passed", "Disabled"})  [unwired: 4 in]
                          n162 = Bundle By Name(cluster=T6 {"Max Current(A)"=FALSE, "Avr Current(A)"=FALSE, "Power"=FALSE, "Time"=FALSE, "Max Current(A) - UpLim"=0.0, "Max Current(A) - MinLim"=0.0, "Max Current(A) - RealValue"=0.0, "Max Current(A) - Result"=FALSE, "Avr Current(A) - UpLim"=0.0, "Avr Current(A) - MinLim"=0.0, "Avr Current(A) - RealValue"=0.0, "Avr Current(A) - Result"=FALSE, "Power- UpLim"=0.0, "Power - MinLim"=0.0, "Power- RealValue"=0.0, "Power - Result"=FALSE, "Time - UpLim"=0.0, "Time - MinLim"=0.0, "Time-RealValue"=0.0, "Time - Result"=FALSE}, "Max Current(A) - RealValue"=w366, "Max Current(A) - Result"=w358, "Avr Current(A) - RealValue"=w364, "Avr Current(A) - Result"=w357, "Power- RealValue"=w361, "Power - Result"=w356, "Time-RealValue"=w360, "Time - Result"=w359) -> (w354:T6)
                          n163 = call "表格组合事件.vi"("颜色"=w427, "字符串"=w428, "Row"=w351, "Col"=2) -> ("结果字符串"=w397:string)  [unwired: 7 in]
                          n164 = call "表格组合事件.vi"("颜色"=w421, "字符串"=w422, "Row"=w351, "Col"=3) -> ("结果字符串"=w396:string)  [unwired: 7 in]
                          n165 = call "表格组合事件.vi"("类型"=enum16{"无", "单格", "整行", "整列"}."无", "字符串"=w408, "Row"=w351, "Col"=1) -> ("结果字符串"=w398:string)  [unwired: 7 in]
                          n166 = call "表格组合事件.vi"("颜色"=w423, "字符串"=w424, "Row"=w351, "Col"=4) -> ("结果字符串"=w395:string)  [unwired: 7 in]
                          n167 = call "表格组合事件.vi"("颜色"=w425, "字符串"=w426, "Row"=w351, "Col"=5) -> ("结果字符串"=w393:string)  [unwired: 7 in]
                          n168 = Build Array(w419, w418, w417, w416) -> (w415:enum16{"Failed", "Passed", "Disabled"}[])
                          n169 = Not Equal To 0?(x=w415) -> (x != 0?=w414:bool[])
                          n170 = And Array Elements(Boolean array=w414) -> (logical AND=w411:bool)
                          n171 = call "CollectAndFormatResult.vi"("Mode"=Mode_ctl."AddResult", "Param/Result"=w354, "Count"=w351) -> ()  [unwired: 8 in, 1 out]
                          n172 = case shown="True" w411 {
                            tunnel: ["NG" "OK"] -> w413
                            tunnel: [u32 16711680 u32 32768] -> w412
                            frame False {
                            }
                            frame True {
                            }
                          }
                          n173 = call "表格组合事件.vi"("颜色"=w412, "字符串"=w413, "Row"=w351, "Col"=6) -> ("结果字符串"=w392:string)  [unwired: 7 in]
                          n174 = Build Array(w398, w397, w396, w395, w393, w392) -> (w394:string[])
                          n175 = Array To Spreadsheet String(delimiter (Tab)="\n", array=w394, 3:"%s" ("格式字符串")) -> (spreadsheet string=w400:string)
                          n176 = Generate User Event(user event=w399, event data cluster=w400) -> ()  [unwired: 2 in, 2 out]
                        }
                        frame #2 {
                          n177 = local read "QR code"() -> (w463:string)
                          n178 = global read "global.vi" "RawDataPath"() -> (w464:path)
                          n179 = String Subset(string=w463, offset (0)=15) -> (substring=w465:string)  [unwired: 1 in]
                          n180 = Build Path(base path=w464, name or relative path=w465) -> (appended path=w473:path)
                          n181 = Increment(x=w456) -> (x+1=w455:i32)
                          n182 = global read "global.vi" "Stop?"() -> (w478:bool)
                          n183 = call <vilib>:"Check if File or Folder Exists.vi"("path"=w473) -> ("file or folder exists?"=w474:bool, "dup path"=w472:path)  [unwired: 8 in, 1 out]
                          n184 = call "SetStripText.vi"() -> ("Now"=w470:timestamp)  [unwired: 9 in, 2 out]
                          n185 = case shown="False" w474 {
                            tunnel: w472 -> [w480 w481]
                            tunnel: [w479 w481] -> w469
                            frame False {
                              n186 = Create Folder(path (use dialog)=w480) -> (created path=w479:path)  [unwired: 2 in, 2 out]
                            }
                            frame True {
                            }
                          }
                          n187 = Format Date/Time String(time format string (%c)="%Y-%m-%d %H-%M-%S" ("时间格式字符串(%c)"), seconds (now)=w470) -> (date/time string=w467:string)  [unwired: 1 in]
                          n188 = Number To Decimal String(number=w455) -> (decimal integer string=w466:string)  [unwired: 1 in]
                          n189 = case shown="False" w478 {
                            tunnel: w477 -> [w483 _]
                            frame False {
                              n190 = Generate User Event(user event=w483, event data cluster="BW\nM56,1") -> ()  [unwired: 2 in, 2 out]
                            }
                            frame True {
                            }
                          }
                          n191 = Concatenate Strings(w467, w466) -> (w468:string)
                          n192 = Build Path(base path=w469, name or relative path=w468) -> (appended path=w461:path)
                          n193 = local read "进度条"() -> (w476:u8)
                          n194 = Increment(x=w476) -> (x+1=w475:u8)
                          n195 = invoke on="波形图" class="WFGraph (strict)" method="Export Image"("FileType"=enum32{"BMP", "EPS", "EMF", "PICT"}."BMP" ("File Type"), "Target"=enum32{"File", "Clipboard"}."File", "Path"=w461, "HideGrid"=TRUE ("Hide Grid"), "Overwrite"=FALSE ("Always Overwrite")) -> ()  [unwired: 3 in, 8 out]
                          n196 = local write "进度条"(w475) -> ()
                        }
                      }
                    }
                    frame True {
                      # "禁用"
                    }
                  }
                }
              }
              frame #2 {
                n197 = Unbundle By Name(w495) -> ("连发打钉次数"=w493:u32)
                n198 = global read "global.vi" "Stop?"() -> (w490:bool)
                n199 = Equal To 0?(x=w493) -> (x = 0?=w491:bool)
                n200 = Compound Arithmetic op=OR(w491, w490) -> (w489:bool)
                n201 = case shown="False" w489 {
                  tunnel: [w496 _] -> w492
                  frame False {
                    n202 = call "提示等待.vi"() -> ("error out"=w496:errorcluster)  [unwired: 11 in]
                  }
                  frame True {
                  }
                }
                n203 = for {
                  N: w493 -> [_]
                  tunnel: w495 -> [w506]
                  tunnel: [w507] -> w494 mode=indexing
                  tunnel: w492 -> [_]
                  tunnel: w488 -> [w501]
                  tunnel: w487 -> [w500]
                  tunnel: w486 -> [w499]
                  tunnel: w485 -> [w498]
                  tunnel: w484 -> [w497]
                  i -> [w504]
                  stop <- w502 stop-if-true
                  n204 = Unbundle By Name(w506) -> ("单发打钉次数"=w505:u32)
                  n205 = global read "global.vi" "Stop?"() -> (w502:bool)
                  n206 = Add(x=w505, y=w504) -> (x+y=w503:u32)
                  n207 = case shown="False" w502 {
                    tunnel: w506 -> [w516 _]
                    tunnel: [w515 _] -> w507
                    tunnel: w504 -> [w514 _]
                    tunnel: w503 -> [w513 _]
                    tunnel: w501 -> [w512 _]
                    tunnel: w500 -> [w511 _]
                    tunnel: w499 -> [w510 _]
                    tunnel: w498 -> [w509 _]
                    tunnel: w497 -> [w508 _]
                    frame False {
                      n208 = stacked-sequence {
                        tunnel: w514 -> [w523 _ w630]
                        tunnel: w516 -> [_ w608 _]
                        tunnel: [_ w574 _] -> w515
                        tunnel: w513 -> [w522 w538 _]
                        tunnel: w512 -> [_ _ w652]
                        tunnel: w511 -> [_ w568 _]
                        tunnel: w510 -> [w520 w545 _]
                        tunnel: w509 -> [_ w543 _]
                        tunnel: w508 -> [_ w540 _]
                        frame #0 {
                          n209 = global read "global.vi" "language"() -> (w519:string)
                          n210 = Increment(x=w523) -> (x+1=w524:i32)
                          n211 = case shown="\"EN\"" w519 {
                            tunnel: ["第%d次连发打钉" ("格式字符串") "Nailing_#%d" ("格式字符串")] -> w518
                            tunnel: ["等待" "Waiting "] -> w517
                            frame "CN", Default {
                            }
                            frame "EN" {
                            }
                          }
                          n212 = Format Into String(format string=w518, w524) -> (resulting string=w527:string)  [unwired: 2 in, 1 out]
                          n213 = call "表格组合事件.vi"("类型"=enum16{"无", "单格", "整行", "整列"}."无", "字符串"=w527, "Row"=w522, "Col"=0) -> ("结果字符串"=w521:string)  [unwired: 7 in]
                          n214 = Concatenate Strings(w517, w527) -> (w528:string)
                          n215 = Generate User Event(user event=w520, event data cluster=w521) -> ()  [unwired: 2 in, 2 out]
                          n216 = call "SetStripText.vi"("Info"=w528) -> ()  [unwired: 8 in, 3 out]
                        }
                        frame #1 {
                          n217 = Greater?(x=w538, y=w568) -> (0:w569:bool)
                          n218 = Unbundle By Name(w608) -> ("最大电流"=w586:bool, "平均电流"=w585:bool, "能量"=w584:bool, "打钉时间"=w583:bool, "触发值"=w542:dbl, "最大电流上限"=w582:dbl, "最大电流下限"=w581:dbl, "平均电流上限"=w580:dbl, "平均电流下限"=w579:dbl, "能量上限"=w578:dbl, "能量下限"=w577:dbl, "时间上限"=w576:dbl, "时间下限"=w575:dbl, "停止值"=w541:dbl, "最大补偿"=w565:dbl, "平均补偿"=w562:dbl, "能量补偿"=w559:dbl, "时间补偿"=w556:dbl, "检查数"=w535:u32, "CurrentType"=w534:enum16{"RMS均方根值", "AVG平均值"})  [unwired: 1 out]
                          n219 = case shown="True" w569 {
                            tunnel: w538 -> [_ w623]
                            tunnel: w568 -> [_ w622]
                            frame False {
                            }
                            frame True {
                              n220 = Subtract(x=w623, y=w622) -> (x-y=w621:u32)
                              n221 = Bundle(w621, 0) -> (w624:cluster{u32, i32})  [unwired: 1 in]
                              n222 = property on="项目" class="Tbl (strict)"("Index Values"=w624) -> ()  [unwired: 2 in, 2 out]
                            }
                          }
                          n223 = global read "GlobalConfigParam.vi" "DebugMode"() -> (w533:bool)
                          n224 = case shown="False" w533 {
                            tunnel: 500 ("采样数") -> [w620 _]
                            tunnel: [w619 _] -> w566
                            tunnel: [w618 _] -> w563
                            tunnel: [w617 _] -> w560
                            tunnel: [w616 _] -> w557
                            tunnel: w543 -> [w614 _]
                            tunnel: w542 -> [w613 _]
                            tunnel: w541 -> [w612 _]
                            tunnel: [w611 _] -> w537
                            tunnel: w535 -> [w610 _]
                            tunnel: w534 -> [w609 _]
                            frame False {
                              n225 = call "电流捕捉 v2.vi"("task/channels in"=w614, "驱动值"=w613, "条件"=1.0, "停止次数"=w610, "采样数"=w620, "CurrentType"=w609, "停止值"=w612) -> ("输出波形"=w611:waveform(dbl), "最大电流"=w619:dbl, "电流值"=w618:dbl, "能量"=w617:dbl, "持续时间"=w616:dbl)  [unwired: 3 in, 1 out]
                            }
                            frame True {
                            }
                          }
                          n226 = Unbundle By Name(w537) -> ("t0"=w573:timestamp)
                          n227 = Format Date/Time String(time format string (%c)="%Y/%m/%d_%H:%M:%S%3u" ("时间格式字符串(%c)"), seconds (now)=w573) -> (date/time string=w571:string)  [unwired: 1 in]
                          n228 = Add(x=w557, y=w556) -> (x+y=w558:dbl)
                          n229 = Add(x=w566, y=w565) -> (x+y=w536:dbl)
                          n230 = Bundle("输出波形"=w537, w536) -> (w539:cluster{"输出波形":waveform(dbl), dbl})  [unwired: 1 in]
                          n231 = Add(x=w563, y=w562) -> (x+y=w564:dbl)
                          n232 = Add(x=w560, y=w559) -> (x+y=w561:dbl)
                          n233 = Generate User Event(user event=w540, event data cluster=w539) -> ()  [unwired: 2 in, 2 out]
                          n234 = call "值比较.vi"("上限"=w576, "下限"=w575, "x"=w558, "s"=w583) -> ("颜色盒"=w600:u32, "值"=w601:string, "结果"=w591:enum16{"Failed", "Passed", "Disabled"})  [unwired: 4 in, 1 out]
                          n235 = call "值比较.vi"("上限"=w582, "下限"=w581, "x"=w536, "s"=w586) -> ("颜色盒"=w602:u32, "值"=w603:string, "结果"=w594:enum16{"Failed", "Passed", "Disabled"})  [unwired: 4 in, 1 out]
                          n236 = call "值比较.vi"("上限"=w578, "下限"=w577, "x"=w561, "s"=w584) -> ("颜色盒"=w598:u32, "值"=w599:string, "结果"=w592:enum16{"Failed", "Passed", "Disabled"})  [unwired: 4 in, 1 out]
                          n237 = call "值比较.vi"("上限"=w580, "下限"=w579, "x"=w564, "s"=w585) -> ("颜色盒"=w596:u32, "值"=w597:string, "结果"=w593:enum16{"Failed", "Passed", "Disabled"})  [unwired: 4 in, 1 out]
                          n238 = call "表格组合事件.vi"("颜色"=w602, "字符串"=w603, "Row"=w538, "Col"=2) -> ("结果字符串"=w554:string)  [unwired: 7 in]
                          n239 = call "表格组合事件.vi"("颜色"=w596, "字符串"=w597, "Row"=w538, "Col"=3) -> ("结果字符串"=w553:string)  [unwired: 7 in]
                          n240 = call "表格组合事件.vi"("类型"=enum16{"无", "单格", "整行", "整列"}."无", "字符串"=w571, "Row"=w538, "Col"=1) -> ("结果字符串"=w555:string)  [unwired: 7 in]
                          n241 = call "表格组合事件.vi"("颜色"=w598, "字符串"=w599, "Row"=w538, "Col"=4) -> ("结果字符串"=w552:string)  [unwired: 7 in]
                          n242 = call "表格组合事件.vi"("颜色"=w600, "字符串"=w601, "Row"=w538, "Col"=5) -> ("结果字符串"=w551:string)  [unwired: 7 in]
                          n243 = Build Array(w594, w593, w592, w591) -> (w590:enum16{"Failed", "Passed", "Disabled"}[])
                          n244 = Not Equal To 0?(x=w590) -> (x != 0?=w589:bool[])
                          n245 = And Array Elements(Boolean array=w589) -> (logical AND=w574:bool)
                          n246 = case shown="True" w574 {
                            tunnel: ["NG" "OK"] -> w588
                            tunnel: [u32 16711680 u32 32768] -> w587
                            frame False {
                            }
                            frame True {
                            }
                          }
                          n247 = call "表格组合事件.vi"("颜色"=w587, "字符串"=w588, "Row"=w538, "Col"=6) -> ("结果字符串"=w550:string)  [unwired: 7 in]
                          n248 = Build Array(w555, w554, w553, w552, w551, w550) -> (w549:string[])
                          n249 = Array To Spreadsheet String(delimiter (Tab)="\n", array=w549, 3:"%s" ("格式字符串")) -> (spreadsheet string=w548:string)
                          n250 = Generate User Event(user event=w545, event data cluster=w548) -> ()  [unwired: 2 in, 2 out]
                        }
                        frame #2 {
                          n251 = local read "QR code"() -> (w647:string)
                          n252 = global read "global.vi" "RawDataPath"() -> (w648:path)
                          n253 = String Subset(string=w647, offset (0)=15) -> (substring=w645:string)  [unwired: 1 in]
                          n254 = Build Path(base path=w648, name or relative path=w645) -> (appended path=w644:path)
                          n255 = Increment(x=w630) -> (x+1=w631:i32)
                          n256 = call <vilib>:"Check if File or Folder Exists.vi"("path"=w644) -> ("file or folder exists?"=w649:bool, "dup path"=w643:path)  [unwired: 8 in, 1 out]
                          n257 = global read "global.vi" "Stop?"() -> (w653:bool)
                          n258 = call "SetStripText.vi"() -> ("Now"=w637:timestamp)  [unwired: 9 in, 2 out]
                          n259 = case shown="False" w649 {
                            tunnel: w643 -> [w655 w656]
                            tunnel: [w654 w656] -> w636
                            frame False {
                              n260 = Create Folder(path (use dialog)=w655) -> (created path=w654:path)  [unwired: 2 in, 2 out]
                            }
                            frame True {
                            }
                          }
                          n261 = Format Date/Time String(time format string (%c)="%Y-%m-%d %H-%M-%S" ("时间格式字符串(%c)"), seconds (now)=w637) -> (date/time string=w634:string)  [unwired: 1 in]
                          n262 = Number To Decimal String(number=w631) -> (decimal integer string=w633:string)  [unwired: 1 in]
                          n263 = case shown="False" w653 {
                            tunnel: w652 -> [w658 _]
                            frame False {
                              n264 = Generate User Event(user event=w658, event data cluster="BW\nM56,1") -> ()  [unwired: 2 in, 2 out]
                            }
                            frame True {
                            }
                          }
                          n265 = Concatenate Strings(w634, w633) -> (w635:string)
                          n266 = local read "进度条"() -> (w651:u8)
                          n267 = Build Path(base path=w636, name or relative path=w635) -> (appended path=w632:path)
                          n268 = Increment(x=w651) -> (x+1=w650:u8)
                          n269 = local write "进度条"(w650) -> ()
                          n270 = invoke on="波形图" class="WFGraph (strict)" method="Export Image"("FileType"=enum32{"BMP", "EPS", "EMF", "PICT"}."BMP" ("File Type"), "Target"=enum32{"File", "Clipboard"}."File", "Path"=w632, "HideGrid"=TRUE ("Hide Grid"), "Overwrite"=FALSE ("Always Overwrite")) -> ()  [unwired: 3 in, 8 out]
                        }
                      }
                    }
                    frame True {
                      # "禁用"
                    }
                  }
                }
              }
              frame #3 {
                w662 = u8 0
                # "结束"
                n271 = Tick Count (ms)() -> (millisecond timer value=w696:u32)
                n272 = call <vilib>:"DAQmx Clear Task.vi"("task in"=w665) -> ()  [unwired: 14 in, 1 out]
                n273 = Subtract(x=w696, y=w695) -> (x-y=w680:u32)
                n274 = Divide(x=w680, y=u32 1000) -> (x/y=w678:dbl)
                n275 = Build Array (concatenate)(w671, w669) -> (w670:bool[])
                n276 = global read "global.vi" "Stop?"() -> (w698:bool)
                n277 = And Array Elements(Boolean array=w670) -> (logical AND=w661:bool)
                n278 = flat-sequence {
                  tunnel: w661 -> [w702]
                  tunnel: [w715] -> w682
                  frame #0 {
                    n279 = call "CollectAndFormatResult.vi"("Mode"=Mode_ctl."ReadData") -> ("Read Data"=w707:string)  [unwired: 10 in]
                    n280 = call "CheckAndControlStateMachine.vi"("Send?"=TRUE, "Mode"=MachineState."Data Ready", "Data formatted csv (comma)"=w707) -> ("error out"=w703:errorcluster)  [unwired: 5 in, 3 out]
                    n281 = call "CheckAndControlStateMachine.vi"("Send?"=TRUE, "OK(T)/NG(F)"=w702, "Mode"=MachineState."OK_NG", "error in (no error)"=w703) -> ("error out"=w700:errorcluster)  [unwired: 4 in, 3 out]
                    n282 = call "CheckAndControlStateMachine.vi"("Mode"=MachineState."WaitMC", "error in (no error)"=w700, "SkipQRcheck"=TRUE) -> ()  [unwired: 5 in, 4 out]
                  }
                  frame #1 {
                    # "#TraceFW reset"
                    n283 = call "CheckAndControlStateMachine.vi"("Mode"=MachineState."Reset") -> ()  [unwired: 7 in, 4 out]
                    n284 = call "CollectAndFormatResult.vi"("Mode"=Mode_ctl."Clear") -> ()  [unwired: 10 in, 1 out]
                  }
                  frame #2 {
                    n285 = call "WaitTime.vi"("wait time(ms)"=u32 500) -> ()  [unwired: 9 in, 2 out]
                  }
                  frame #3 {
                    n286 = local read "项目"() -> (w716:string[][])
                    n287 = call "2D数组转1D数组.vi"("列索引"=2, "行索引"=0, "2D表格"=w716) -> ("1D表格"=w715:string[])  [unwired: 8 in]
                  }
                }
                n288 = Format Value(format string="%.2f秒" ("格式字符串"), value (0)=w678) -> (output string=w672:string)  [unwired: 1 in]
                n289 = case shown="False" w698 {
                  tunnel: w661 -> [w732 _]
                  tunnel: [w730 "已取消测试"] -> w694
                  tunnel: [w731 w753] -> w673
                  tunnel: w672 -> [w729 _]
                  tunnel: w667 -> [w728 _]
                  tunnel: [w721 w753] -> w664
                  tunnel: [w720 T2 {"Text Color"=0, "Background Color"=16776960} ("文本.文本颜色")] -> w663
                  frame False {
                    # "#TraceForward send M to reset start"
                    n290 = case shown="False" w732 {
                      tunnel: ["FAIL" "PASS"] -> w731
                      tunnel: ["BT\nM53,0\nM54,1" "BT\nM53,1\nM54,0"] -> w717
                      tunnel: ["不良品数" ("key") "良品数" ("key")] -> w723
                      tunnel: [w739 w748] -> w722
                      tunnel: [w736 w745] -> w721
                      tunnel: [T2 {"Text Color"=16777225, "Background Color"=16711680} ("文本.文本颜色") T2 {"Text Color"=16777225, "Background Color"=32768} ("文本.文本颜色")] -> w720
                      frame False {
                        n291 = global read "global.vi" "language"() -> (w737:string)
                        n292 = case shown="\"EN\"" w737 {
                          tunnel: ["测试失败" ("Title") "TEST FAILED" ("Title")] -> w736
                          frame "CN", Default {
                          }
                          frame "EN" {
                          }
                        }
                        n293 = call "Fail++.vi"() -> ("数值"=w739:u32)  [unwired: 11 in]
                      }
                      frame True {
                        n294 = global read "global.vi" "language"() -> (w746:string)
                        n295 = case shown="\"EN\"" w746 {
                          tunnel: ["测试通过" ("Title") "TEST PASSED" ("Title")] -> w745
                          frame "CN", Default {
                          }
                          frame "EN" {
                          }
                        }
                        n296 = call "Pass++.vi"() -> ("数值"=w748:u32)  [unwired: 11 in]
                      }
                    }
                    n297 = global read "global.vi" "language"() -> (w719:string)
                    n298 = Generate User Event(user event=w728, event data cluster=w717) -> ()  [unwired: 2 in, 2 out]
                    n299 = global read "global.vi" "ConfigPath"() -> (w724:path)
                    n300 = call <vilib>:"Open Config Data.vi"("configuration file path"=w724) -> ("refnum"=w725:T7)  [unwired: 8 in, 2 out]
                    n301 = case shown="\"EN\"" w719 {
                      tunnel: ["测试结束，用时" ("格式字符串") "Test Complete, Test Time is " ("格式字符串")] -> w718
                      frame "CN", Default {
                      }
                      frame "EN" {
                      }
                    }
                    n302 = local read "型号"() -> (w727:string)
                    n303 = call <vilib>:"Write Key (U32).vi"("section"=w727, "value"=w722, "key"=w723, "refnum"=w725) -> ("refnum out"=w726:T7)  [unwired: 5 in, 2 out]
                    n304 = call <vilib>:"Close Config Data.vi"("refnum"=w726) -> ()  [unwired: 9 in, 2 out]
                    n305 = Concatenate Strings(w718, w729) -> (w730:string)
                  }
                  frame True {
                    n306 = global read "global.vi" "language"() -> (w754:string)
                    n307 = case shown="\"EN\"" w754 {
                      tunnel: ["已取消" "Cancel" ("格式字符串")] -> w753
                      frame "CN", Default {
                      }
                      frame "EN" {
                      }
                    }
                  }
                }
                n308 = call "SetStripText.vi"("Info"=w694) -> ("time"=w674:string, "Now"=w681:timestamp)  [unwired: 8 in, 1 out]
                n309 = property on="Title" class="Str"("Value"=w664, "Text.TextColors"=w663) -> ()  [unwired: 2 in, 2 out]
                n310 = local read "QR code"() -> (w659:string)
                n311 = local read "型号"() -> (w683:string)
                n312 = global read "global.vi" "ReportPath"() -> (w697:path)
                n313 = Format Date/Time String(time format string (%c)="%Y-%m" ("时间格式字符串(%c)"), seconds (now)=w681) -> (date/time string=w692:string)  [unwired: 1 in]
                n314 = Concatenate Strings(w683, "_" ("字符串"), w692, ".xls" ("字符串")) -> (w690:string)
                n315 = Build Array (concatenate)(w659, w674, w673, w672, w682) -> (w676:string[])
                n316 = Build Path(base path=w697, name or relative path=w690) -> (appended path=w689:path)
                n317 = Build Array(w676) -> (w675:string[][])
                n318 = call <vilib>:"Check if File or Folder Exists.vi"("path"=w689) -> ("file or folder exists?"=w685:bool, "dup path"=w686:path)  [unwired: 8 in, 1 out]
                n319 = Build Array (concatenate)(string[][] [["", "", "", "", "Item 1", "", "", "", "", "Item 2", "", "", "", "", "Item 3", "", "", "", "", "Item 4", "", "", "", "", "Item 5", "", "", "", "", "Item 6", "", "", "", "", "Item 7", "", "", "", "", "Item 8", "", "", "", "", "Item 9", "", "", "", "", "Item 10", "", "", "", "", "Item 11", "", "", "", "", "Item 12", "", "", "", "", "Item 13", "", "", "", "", "Item 14", "", "", "", "", "Item 15", "", "", "", "", "Item 16", "", "", "", "", "Item 17", "", "", "", "", "Item 18", "", "", "", "", "Item 19", "", "", "", "", "Item 20", "", "", "", ""], ["QR Code", "Date Time", "Test Result", "Test Time", "Peak amps", "RMS amps", "Power", "Time", "Result", "Peak amps", "RMS amps", "Power", "Time", "Result", "Peak amps", "RMS amps", "Power", "Time", "Result", "Peak amps", "RMS amps", "Power", "Time", "Result", "Peak amps", "RMS amps", "Power", "Time", "Result", "Peak amps", "RMS amps", "Power", "Time", "Result", "Peak amps", "RMS amps", "Power", "Time", "Result", "Peak amps", "RMS amps", "Power", "Time", "Result", "Peak amps", "RMS amps", "Power", "Time", "Result", "Peak amps", "RMS amps", "Power", "Time", "Result", "Peak amps", "RMS amps", "Power", "Time", "Result", "Peak amps", "RMS amps", "Power", "Time", "Result", "Peak amps", "RMS amps", "Power", "Time", "Result", "Peak amps", "RMS amps", "Power", "Time", "Result", "Peak amps", "RMS amps", "Power", "Time", "Result", "Peak amps", "RMS amps", "Power", "Time", "Result", "Peak amps", "RMS amps", "Power", "Time", "Result", "Peak amps", "RMS amps", "Power", "Time", "Result", "Peak amps", "RMS amps", "Power", "Time", "Result", "Peak amps", "RMS amps", "Power", "Time", "Result"]] ("数组"), w675) -> (w688:string[][])
                n320 = global write "global.vi" "Start"(FALSE ("Start")) -> ()
                n321 = property on="Exit" class="Bool"("DisabledEnum"=w662) -> ()  [unwired: 2 in, 2 out]
                n322 = property on="开始" class="Bool"("DisabledEnum"=w662) -> ()  [unwired: 2 in, 2 out]
                n323 = property on="设置" class="Bool"("DisabledEnum"=w662) -> ()  [unwired: 2 in, 2 out]
                n324 = property on="清零" class="Bool"("DisabledEnum"=w662) -> ()  [unwired: 2 in, 2 out]
                n325 = Select(t=w675, s=w685, f=w688) -> (s? t:f=w687:string[][])
                n326 = property on="Stop" class="Bool"("DisabledEnum"=2) -> ()  [unwired: 2 in, 2 out]
                n327 = property on="型号" class="CmbBox"("DisabledEnum"=w662) -> ()  [unwired: 2 in, 2 out]
                n328 = call <vilib>:"Write To Spreadsheet File (string).vi"("append to file? (new file:F)"=w685, "2D data"=w687, "file path (dialog if empty)"=w686) -> ()  [unwired: 5 in, 1 out]
              }
            }
          }
        }
      }
      n329 = Create User Event(user event datatype=w126) -> (user event=w125:refnum<user-event>)  [unwired: 1 in, 1 out]
      n330 = global read "global.vi" "Modbus"() -> (w110:string)
      n331 = register-events(w125, w121, w120, w118, w116, w115) -> (reference out=w128:refnum<event-registration>, error out=w123:errorcluster)  [unwired: 2 in]
      n332 = call-poly <vilib>:"Create Modbus Instance.vi"("serial type"=enum16{"RTU", "ASCII"}."RTU", "parity (even)"=w108, "unit ID"=u8 1, "baud rate"=u32 9600, "VISA resource name"=w110) -> ("error out"=w105:errorcluster, "serial master instance"=w104:refnum<class "Modbus Master.lvclass">)  [unwired: 5 in]
      n333 = Generate User Event(user event=w125, event data cluster=w122, error in=w123) -> (user event out=w124:refnum<user-event>)  [unwired: 1 in, 1 out]
      n334 = while {
        tunnel: w128 -> [w765]
        tunnel: w120 -> [w764]
        tunnel: w124 -> [w762]
        tunnel: w121 -> [w761]
        tunnel: w116 -> [w760]
        tunnel: w113 -> [w759]
        stop <- FALSE stop-if-true
        n335 = event shown="[0] Timeout" {
          selector: w765 -> [_ _ _ _ _ _ _ _ _ _ _ _ _ _ _]
          dyn-events: _ -> [_ _ _ _ _ _ _ _ _ _ _ _ _ _ _]
          timeout: 70 -> [_ _ _ _ _ _ _ _ _ _ _ _ _ _ _]
          tunnel: w764 -> [_ _ _ w907 _ _ _ _ _ _ _ _ _ _ _]
          tunnel: w762 -> [_ _ _ _ _ _ _ _ _ _ _ _ w1077 _ _]
          tunnel: w761 -> [w768 _ _ w884 _ _ _ _ _ _ _ _ _ _ _]
          tunnel: w760 -> [w769 _ _ _ _ _ _ _ _ _ _ _ _ _ _]
          tunnel: w759 -> [_ _ _ w877 _ _ _ _ _ _ _ _ _ _ _]
          event Timeout {
            n336 = event-data() -> ()  [unwired: 1 in, 3 out]
            n337 = global read "GlobalConfigParam.vi" "DebugMode"() -> (w767:bool)
            n338 = case shown="False" w767 {
              tunnel: w769 -> [w804 _]
              tunnel: w768 -> [w786 _]
              frame False {
                # "#TraceFW read PLC error"
                n339 = global read "global.vi" "PLC"() -> (w803:string)
                n340 = call "SerialOpen.vi"("Timeout"=u32 200, "parity"=enum16{"None", "Odd", "Even", "Mark", "Space"}."None", "Data Bits"=u16 8, "Baud Rate"=u32 19200, "Port"=w803) -> ("error out"=w799:errorcluster, "Port out"=w800:refnum<visa-resource-name>)  [unwired: 5 in]
                n341 = call "FX232_485_BRWR.vi"("延时"=u8 50, "PLC站号"=u8 1, "error in (no error)"=w799, "地址"="X10", "命令"="WR", "Port"=w800) -> ("error out"=w794:errorcluster, "Value"=w796:string, "PortOut"=w795:refnum<visa-resource-name>)  [unwired: 2 in, 1 out]
                n342 = call "FX232_485_BRWR.vi"("延时"=u8 50, "数量"=u8 5, "PLC站号"=u8 1, "error in (no error)"=w794, "地址"="M51", "命令"="BR", "Port"=w795) -> ("error out"=w783:errorcluster, "Value"=w790:string, "PortOut"=w785:refnum<visa-resource-name>)  [unwired: 1 in, 1 out]
                n343 = control-ref of="PLC连接状态"() -> (w787:refnum<vi>)
                n344 = call "FX232_485_BRWR.vi"("延时"=u8 50, "数量"=u8 1, "PLC站号"=u8 1, "error in (no error)"=w783, "地址"="M500", "命令"="BR", "Port"=w785) -> ("error out"=w782:errorcluster, "Value"=w778:string, "PortOut"=w784:refnum<visa-resource-name>)  [unwired: 1 in, 1 out]
                n345 = VISA Close(VISA resource name=w784, error in (no error)=w782) -> (error out=w789:errorcluster)
                n346 = Unbundle By Name(w789) -> ("status"=w788:bool)
                n347 = call "ValueChangeTrigger.vi"("新值"=w788, "控件引用"=w787) -> ()  [unwired: 10 in]
                n348 = case shown="No Error" w789 {
                  tunnel: w804 -> [w824 w844]
                  tunnel: w796 -> [w816 _]
                  tunnel: w790 -> [w813 _]
                  tunnel: w786 -> [w811 _]
                  tunnel: w778 -> [w808 _]
                  frame No Error {
                    # "#TraceFW if there is any issue from apptrace"
                    n349 = call "Hex2Bits.vi"("Value"=w816) -> ("Bits"=w815:bool[])  [unwired: 4 in]
                    n350 = call "Bits2Bools.vi"("Bits"=w813) -> ("Bools"=w814:bool[])  [unwired: 4 in]
                    n351 = property on="Error message" class="Str"() -> ("Text.Text"=w812:string)  [unwired: 2 in, 2 out]
                    n352 = Index Array(array=w815, index #1=3 ("索引")) -> (element #1=w820:bool, element #2=w821:bool)  [unwired: 1 in]
                    n353 = Index Array(array=w814, index #2=4 ("索引")) -> (element #1=w817:bool, element #2=w818:bool)  [unwired: 1 in]
                    n354 = Compound Arithmetic op=OR(w818, invert w821) -> (w823:bool)
                    n355 = Equal?(x=w808, y="1") -> (x = y?=w805:bool)
                    n356 = call "ConvertErrorToPLCMBits.vi"("Error message"=w812) -> ("PLC message"=w809:string, "Send?"=w810:bool)  [unwired: 9 in]
                    n357 = Or(x=w823, y=w805) -> (x .or. y?=w806:bool)
                    n358 = case shown="False" w817 {
                      selector: w817 -> [_ w834]
                      frame False {
                      }
                      frame True {
                        n359 = global write "global.vi" "Start"(w834) -> ()
                      }
                    }
                    n360 = case shown="True" w806 {
                      selector: w806 -> [_ w839]
                      frame False {
                      }
                      frame True {
                        n361 = global write "global.vi" "Stop?"(w839) -> ()
                        n362 = call "CheckAndControlStateMachine.vi"("Mode"=MachineState."Stop") -> ("error out"=w837:errorcluster)  [unwired: 7 in, 3 out]
                        n363 = call <vilib>:"Clear Errors.vi"("error in (no error)"=w837) -> ("error out"=w836:errorcluster)  [unwired: 5 in, 1 out]
                        n364 = call "CheckAndControlStateMachine.vi"("Mode"=MachineState."Reset", "error in (no error)"=w836) -> ()  [unwired: 6 in, 4 out]
                      }
                    }
                    n365 = case shown="True" w820 {
                      selector: w820 -> [_ w832]
                      tunnel: w824 -> [_ w833]
                      frame False {
                      }
                      frame True {
                        (unwired) MachineState."Stop" ("Mode")
                        # "#TraceFW\nReset send stop"
                        n366 = Generate User Event(user event=w833, event data cluster=w832) -> (error out=w828:errorcluster)  [unwired: 2 in, 1 out]
                        n367 = call "CheckAndControlStateMachine.vi"("error in (no error)"=w828) -> ("error out"=w830:errorcluster)  [unwired: 7 in, 3 out]
                        n368 = call <vilib>:"Clear Errors.vi"("error in (no error)"=w830) -> ("error out"=w829:errorcluster)  [unwired: 5 in, 1 out]
                        n369 = call "CheckAndControlStateMachine.vi"("Mode"=MachineState."Reset", "error in (no error)"=w829) -> ()  [unwired: 6 in, 4 out]
                      }
                    }
                    n370 = case shown="True" w810 {
                      selector: w810 -> [_ w825]
                      tunnel: w811 -> [_ w827]
                      tunnel: w809 -> [_ w826]
                      frame False {
                      }
                      frame True {
                        # "#TraceFW send error to PLC"
                        n371 = global write "global.vi" "Stop?"(w825) -> ()
                        n372 = Generate User Event(user event=w827, event data cluster=w826) -> ()  [unwired: 2 in, 2 out]
                      }
                    }
                  }
                  frame Error {
                    # "#TraceFW\nReset send stop"
                    n373 = Generate User Event(user event=w844, event data cluster=TRUE ("event data")) -> (error out=w842:errorcluster)  [unwired: 2 in, 1 out]
                    n374 = call "CheckAndControlStateMachine.vi"("Mode"=MachineState."Stop", "error in (no error)"=w842) -> ("error out"=w841:errorcluster)  [unwired: 6 in, 3 out]
                    n375 = call <vilib>:"Clear Errors.vi"("error in (no error)"=w841) -> ("error out"=w840:errorcluster)  [unwired: 5 in, 1 out]
                    n376 = call "CheckAndControlStateMachine.vi"("Mode"=MachineState."Reset", "error in (no error)"=w840) -> ()  [unwired: 6 in, 4 out]
                  }
                }
              }
              frame True {
              }
            }
          }
          event "PLC连接状态": Value Change {
            n377 = event-data() -> ("NewVal"=w847:bool)  [unwired: 1 in, 1 out]
            n378 = case shown="True" w847 {
              frame False {
              }
              frame True {
                n379 = global read "GlobalConfigParam.vi" "DebugMode"() -> (w848:bool)
                n380 = case shown="False" w848 {
                  frame False {
                    n381 = vi-ref "错误设备提示.vi"() -> (w864:refnum<vi>)
                    n382 = property class="VI Interface Type 0"(reference=w864) -> (reference out=w852:refnum<vi>, "Name"=w863:string)  [unwired: 1 in, 1 out]
                    n383 = Open VI Reference(type specifier VI Refnum (for type only)=w852, vi path=w863, options=128 ("选项")) -> (vi reference=w851:refnum<vi>, error out=w853:errorcluster)  [unwired: 3 in]
                    n384 = global read "global.vi" "language"() -> (w861:string)
                    n385 = case shown="\"EN\"" w861 {
                      tunnel: ["遇到以下错误，将无法正常测试：" ("Titre") "Found Fllowing Error Messages,\nThe Software Cannot Start Testing:" ("Titre")] -> w860
                      tunnel: ["与PLC连接断开" ("source") "Disconnect from PLC" ("source")] -> w859
                      frame "CN", Default {
                      }
                      frame "EN" {
                      }
                    }
                    n386 = Bundle("status"=TRUE, "code"=0, "source"=w859) -> (w855:errorcluster)  [unwired: 1 in]
                    n387 = Build Array(w855) -> (w854:errorcluster[])
                    n388 = call-by-ref "开始异步调用"(reference=w851, error in=w853, "Titre"=w860, "错误数组"=w854, "设备列表"=string[] ["PLC"]) -> (reference out=w849:refnum<vi>, error out=w850:errorcluster)  [unwired: 7 in, 2 out]
                    n389 = Close Reference(reference=w849, error in (no error)=w850) -> ()  [unwired: 1 out]
                  }
                  frame True {
                  }
                }
              }
            }
          }
          event User Event {
            n390 = event-data() -> ()  [unwired: 1 in, 3 out]
            n391 = global read "global.vi" "Start"() -> (w869:bool)
            n392 = case shown="True" w869 {
              frame False {
              }
              frame True {
                n393 = flat-sequence {
                  frame #0 {
                    n394 = global write "global.vi" "Stop?"(TRUE) -> ()
                  }
                  frame #1 {
                    n395 = call "WaitTime.vi"("wait time(ms)"=u32 1000) -> ()  [unwired: 9 in, 2 out]
                    n396 = property on="项目" class="Tbl (strict)"("Active Cell"=cluster{"Row":i32, "Column":i32} {"Row"=-2, "Column"=-2} ("活动单元格:活动单元格"), "Cell BG Color"=u32 16777225, "Value"=string[][] [], "Index Values"=cluster{"Row":u32, "Column":u32} {"Row"=0, "Column"=0} ("索引值")) -> ()  [unwired: 2 in, 2 out]
                  }
                  frame #2 {
                    n397 = global write "global.vi" "Start"(TRUE) -> ()
                  }
                }
              }
            }
          }
          event "型号": Value Change {
            w885 = TRUE
            n398 = event-data() -> ("OldVal"=w880:string, "NewVal"=w879:string)  [unwired: 1 in]
            n399 = global read "global.vi" "ConfigPath"() -> (w906:path)
            n400 = Generate User Event(user event=w907, event data cluster=TRUE ("事件数据")) -> ()  [unwired: 2 in, 2 out]
            n401 = call <vilib>:"Open Config Data.vi"("configuration file path"=w906) -> ("refnum"=w881:T7)  [unwired: 8 in, 2 out]
            n402 = property on="项目" class="Tbl (strict)"("Active Cell"=cluster{"Row":i32, "Column":i32} {"Row"=-2, "Column"=-2} ("活动单元格:活动单元格"), "Cell BG Color"=u32 16777225, "Value"=string[][] [] ("项目")) -> ()  [unwired: 2 in, 2 out]
            n403 = local write "波形图"(waveform(dbl) {"t0"=timestamp(0 s since 1904-01-01), "dt"=1.0, "Y"=[]} ("Waveform")) -> ()
            n404 = Not Equal?(x=w880, y=w879) -> (x != y?=w897:bool)
            n405 = case shown="False" w897 {
              tunnel: w881 -> [w932 w937]
              tunnel: [w932 w936] -> w898
              tunnel: w879 -> [_ w933]
              frame False {
              }
              frame True {
                n406 = call <vilib>:"Write Key (String).vi"("section"="COMMON", "value"=w933, "key"="LastModel", "refnum"=w937) -> ("refnum out"=w936:T7)  [unwired: 5 in, 2 out]
              }
            }
            n407 = property on="Title" class="Str"("Value"="" ("Title"), "Text.TextColors"=T2 {"Text Color"=0, "Background Color"=16777225} ("文本.文本颜色")) -> ()  [unwired: 2 in, 2 out]
            n408 = global read "global.vi" "ConfigPara"() -> (w900:T9)
            n409 = vi-ref "global.vi"() -> (w902:refnum<vi>)
            n410 = call "ReadConfigToCluster.vi"("簇名"="Para" ("section"), "VI引用"=w902, "ConfigInfo"=w900, "section"=w879, "refnum"=w898) -> ("error out"=w878:errorcluster, "refnum out"=w894:refnum<k1>)  [unwired: 5 in]
            n411 = call <vilib>:"Read Key (String).vi"("section"=w879, "default value"="0", "key"="良品数", "refnum"=w894) -> ("value"=w888:string, "refnum out"=w893:T7)  [unwired: 4 in, 2 out]
            n412 = call <vilib>:"Read Key (String).vi"("section"=w879, "default value"="0", "key"="不良品数", "refnum"=w893) -> ("value"=w887:string, "refnum out"=w886:T7)  [unwired: 4 in, 2 out]
            n413 = call "Fail++.vi"("字符串"=w887, "reset"=w885) -> ()  [unwired: 9 in, 1 out]
            n414 = call "Pass++.vi"("字符串"=w888, "reset"=w885) -> ()  [unwired: 9 in, 1 out]
            n415 = case shown="No Error" w878 {
              tunnel: w877 -> [w908 _]
              frame No Error {
                n416 = global read "global.vi" "Para"() -> (w913:T8)
                n417 = Unbundle By Name(w913) -> ("最大电流"=w912:bool, "平均电流"=w911:bool, "能量"=w910:bool, "打钉时间"=w909:bool)
                n418 = Build Array(w912, w911, w910, w909) -> (w914:bool[])
                n419 = for {
                  tunnel: w914 -> [w921] mode=indexing
                  tunnel: w908 -> [w916] mode=indexing
                  i -> [w923]
                  n420 = Add(x=2, y=w923) -> (x+y=w919:i32)
                  n421 = Select(t=w916, s=w921, f=u32 0) -> (s? t:f=w917:u32)
                  n422 = Bundle(-1, w919) -> (w918:cluster{i32, i32})  [unwired: 1 in]
                  n423 = property on="项目" class="Tbl (strict)"("Active Cell"=w918, "Width"=w917) -> ()  [unwired: 2 in, 2 out]
                }
              }
              frame Error {
              }
            }
            n424 = call <vilib>:"Close Config Data.vi"("refnum"=w886) -> ("error out"=w883:errorcluster)  [unwired: 9 in, 1 out]
            n425 = case shown="No Error" w883 {
              tunnel: w884 -> [w931 _]
              frame No Error {
                n426 = global read "global.vi" "Para"() -> (w930:T8)
                n427 = Unbundle By Name(w930) -> ("单发打钉次数"=w927:u32, "连发打钉次数"=w925:u32)
                n428 = Format Into String(format string="WT\n%s,%x\n%s,%x" ("格式字符串"), "D500" ("地址"), w927, "D502" ("地址"), w925) -> (resulting string=w924:string)  [unwired: 2 in, 1 out]
                n429 = Generate User Event(user event=w931, event data cluster=w924) -> ()  [unwired: 2 in, 2 out]
              }
              frame Error {
              }
            }
          }
          event "Exit": Value Change; Panel Close {
            n430 = event-data() -> ()  [unwired: 1 in, 3 out]
            n431 = flat-sequence {
              tunnel: [w939] -> w938
              tunnel: w938 -> [_]
              frame #0 {
                # "#TraceFW"
                n432 = call "CloseQueueHostConnection.vi"() -> ("error out"=w940:errorcluster)  [unwired: 11 in]
                n433 = call "CloseLog.vi"("error in (no error)"=w940) -> ("error out"=w939:errorcluster)  [unwired: 10 in]
              }
              frame #1 {
                n434 = disable-structure shown="Default" {
                  frame condition #0 {
                    n435 = Quit LabVIEW() -> ()  [unwired: 1 in]
                  }
                  frame condition #1 (active) {
                    n436 = Stop() -> ()  [unwired: 1 in]
                  }
                }
              }
            }
          }
          event Panel Close? {
            n437 = event-data() -> ()  [unwired: 1 in, 4 out]
            n438 = flat-sequence {
              tunnel: [FALSE] -> w941
              frame #0 {
                n439 = global write "global.vi" "Stop?"(TRUE) -> ()
              }
              frame #1 {
                n440 = call "WaitTime.vi"("wait time(ms)"=u32 100) -> ()  [unwired: 9 in, 2 out]
              }
              frame #2 {
              }
            }
            n441 = event-data("Discard?"=w941) -> ()  [unwired: 1 in, 1 out]
          }
          event "Stop": Value Change {
            n442 = event-data() -> ("NewVal"=w945:bool)  [unwired: 1 in]
            n443 = case shown="True" w945 {
              selector: w945 -> [_ w946]
              frame False {
              }
              frame True {
                n444 = global write "global.vi" "Stop?"(w946) -> ()
              }
            }
          }
          event User Event {
            w956 = 500.0 ("y")
            w951 = 10.0 ("y")
            n445 = event-data() -> ("Waveform"=w947:waveform(dbl), "最大电流"=w948:dbl)  [unwired: 1 in, 4 out]
            n446 = Multiply(x=w948, y=1.25) -> (x*y=w952:dbl)
            n447 = Divide(x=w952, y=w951) -> (x/y=w949:dbl)
            n448 = Round Toward +Infinity(x=w949) -> (ceil(x): smallest int >= x=w950:dbl)
            n449 = Multiply(x=w950, y=w951) -> (x*y=w955:dbl)
            n450 = Greater?(x=w955, y=w956) -> (0:w954:bool)
            n451 = Select(t=w956, s=w954, f=w955) -> (s? t:f=w957:dbl)
            n452 = property on="波形图" class="WFGraph (strict)"("Value"=w947, "YScale.Maximum"=w957) -> ()  [unwired: 2 in, 2 out]
          }
          event User Event {
            n453 = event-data() -> ("发送"=w959:string)  [unwired: 1 in]
            n454 = global read "GlobalConfigParam.vi" "DebugMode"() -> (w958:bool)
            n455 = case shown="False" w958 {
              tunnel: w959 -> [w967 _]
              frame False {
                n456 = Spreadsheet String To Array(delimiter (Tab)="\n", format string="%s" ("格式字符串"), spreadsheet string=w967, array type (2D Dbl)=string[] []) -> (array=w971:string[])
                n457 = global read "global.vi" "PLC"() -> (w977:string)
                n458 = Delete From Array(array=w971, index=0 ("索引")) -> (deleted portion=w972:string, array with subset deleted=w973:string[])  [unwired: 1 in]
                n459 = call "SerialOpen.vi"("Timeout"=u32 200, "termination char"=u8 1, "parity"=enum16{"None", "Odd", "Even", "Mark", "Space"}."None", "Data Bits"=u16 8, "Baud Rate"=u32 19200, "Port"=w977) -> ("error out"=w965:errorcluster, "Port out"=w966:refnum<visa-resource-name>)  [unwired: 4 in]
                n460 = case shown="\"BW\", \"WW\", Default" w972 {
                  selector: w972 -> [w985 w999]
                  tunnel: w966 -> [w986 w1000]
                  tunnel: w973 -> [w983 w998]
                  tunnel: [w982 w997] -> w964
                  tunnel: w965 -> [w980 w995]
                  tunnel: [w981 w996] -> w963
                  frame "BT", "WT" {
                    n461 = for {
                      tunnel: w983 -> [w992] mode=indexing
                      tunnel: [w994] -> w984 mode=indexing if=w987
                      n462 = Match Pattern(string=w992, regular expression="," ("正则表达式")) -> (before substring=w990:string, after substring=w989:string, offset past match=w988:i32)  [unwired: 1 in, 1 out]
                      n463 = Greater Or Equal To 0?(x=w988) -> (x >= 0?=w987:bool)
                      n464 = Bundle(cluster=cluster{"地址":string, "值":string} {"地址"="", "值"=""} ("簇"), "地址"=w990, "值"=w989) -> (w994:cluster{"地址":string, "值":string})
                    }
                    n465 = call "FX232_485_BTWT.vi"("延时"=u8 50, "PLC站号"=u8 1, "error in (no error)"=w980, "地址值"=w984, "命令"=w985, "Port"=w986) -> ("error out"=w982:errorcluster, "PortOut"=w981:refnum<visa-resource-name>)  [unwired: 2 in, 2 out]
                  }
                  frame "BW", "WW", Default {
                    n466 = for {
                      tunnel: w1000 -> [w1010]
                      tunnel: w999 -> [w1009]
                      tunnel: w998 -> [w1007] mode=indexing
                      shift-right: [w1003] -> w997
                      shift-left: w995 -> [w1002]
                      tunnel: [w1001] -> w996
                      n467 = Match Pattern(string=w1007, regular expression="," ("正则表达式")) -> (before substring=w1006:string, after substring=w1005:string, offset past match=w1004:i32)  [unwired: 1 in, 1 out]
                      n468 = case shown="0.." w1004 {
                        tunnel: w1010 -> [w1011 w1021]
                        tunnel: w1009 -> [_ w1020]
                        tunnel: w1006 -> [_ w1019]
                        tunnel: w1005 -> [_ w1018]
                        tunnel: [w1012 w1017] -> w1003
                        tunnel: w1002 -> [w1012 w1016]
                        tunnel: [w1011 w1015] -> w1001
                        frame -1, Default {
                        }
                        frame 0.. {
                          n469 = call "FX232_485_BWWW.vi"("值"=w1018, "延时"=u8 50, "PLC站号"=u8 1, "error in (no error)"=w1016, "地址"=w1019, "命令"=w1020, "Port"=w1021) -> ("error out"=w1017:errorcluster, "PortOut"=w1015:refnum<visa-resource-name>)  [unwired: 1 in, 2 out]
                        }
                      }
                    }
                  }
                }
                n470 = VISA Close(VISA resource name=w963, error in (no error)=w964) -> ()  [unwired: 1 out]
              }
              frame True {
              }
            }
          }
          event "开始": Value Change {
            n471 = event-data() -> ()  [unwired: 1 in, 6 out]
            n472 = global write "global.vi" "Start"(TRUE ("Start")) -> ()
          }
          event User Event {
            n473 = event-data() -> ()  [unwired: 1 in, 5 out]
            n474 = global read "GlobalConfigParam.vi" "DebugMode"() -> (w1023:bool)
            n475 = case shown="False" w1023 {
              frame False {
                n476 = global read "global.vi" "PLC"() -> (w1036:string)
                n477 = disable-structure shown="Default" {
                  disable-tunnel: [FALSE FALSE] -> w1024
                  frame condition #0 (active) {
                  }
                  frame condition #1 {
                  }
                }
                n478 = call "SerialOpen.vi"("Timeout"=u32 200, "termination char"=u8 1, "parity"=enum16{"None", "Odd", "Even", "Mark", "Space"}."None", "Data Bits"=u16 8, "Baud Rate"=u32 19200, "Port"=w1036) -> ("error out"=w1035:errorcluster, "Port out"=w1037:refnum<visa-resource-name>)  [unwired: 4 in]
                n479 = call "FX232_485_RRRSTT.vi"("延时"=u8 50, "PLC站号"=u8 1, "error in (no error)"=w1035, "值"="ABC", "命令"="TT", "Port"=w1037) -> ("error out"=w1031:errorcluster, "PortOut"=w1032:refnum<visa-resource-name>)  [unwired: 2 in, 2 out]
                n480 = call "查找DAQ.vi"("允许仿真"=w1024) -> ("error out"=w1045:errorcluster, "DAQmx设备名"=w1044:tag)  [unwired: 9 in]
                n481 = VISA Close(VISA resource name=w1032, error in (no error)=w1031) -> (error out=w1030:errorcluster)
                n482 = Concatenate Strings(w1044, "/ai5" ("字符串")) -> (w1047:string)
                n483 = global write "global.vi" "输入通道"(w1047) -> ()
                n484 = Build Array(w1045, w1030) -> (w1043:errorcluster[])
                n485 = global read "global.vi" "language"() -> (w1040:string)
                n486 = Unbundle By Name(w1030) -> ("status"=→"PLC连接状态":bool)
                n487 = case shown="\"EN\"" w1040 {
                  tunnel: ["遇到以下错误，将无法正常测试：" ("Titre") "Found Fllowing Error Messages,\nThe Software Cannot Start Testing:" ("Titre")] -> w1039
                  frame "CN", Default {
                  }
                  frame "EN" {
                  }
                }
                n488 = call "错误设备提示.vi"("Titre"=w1039, "错误数组"=w1043, "设备列表"=string[] ["DAQ", "PLC"]) -> ("error out"=w1041:errorcluster)  [unwired: 7 in, 1 out]
                n489 = call <vilib>:"Clear Errors.vi"("error in (no error)"=w1041) -> ()  [unwired: 5 in, 2 out]
              }
              frame True {
              }
            }
          }
          event "清零": Value Change {
            n490 = event-data() -> ()  [unwired: 1 in, 6 out]
            n491 = disable-structure shown="Enabled" {
              disable-tunnel: [w1060 TRUE] -> w1059
              frame Disabled {
                n492 = Two Button Dialog(message="是否将计数清零？" ("消息"), 1:"否" ("F按钮名称（“取消”）"), 2:"是" ("T按钮名称（“确定”）")) -> (T button?=w1060:bool)
              }
              frame Enabled {
              }
            }
            n493 = case shown="True" w1059 {
              frame False {
              }
              frame True {
                w1074 = TRUE ("reset")
                n494 = call "Fail++.vi"("reset"=w1074) -> ()  [unwired: 10 in, 1 out]
                n495 = call "Pass++.vi"("reset"=w1074) -> ()  [unwired: 10 in, 1 out]
                n496 = global read "global.vi" "ConfigPath"() -> (w1071:path)
                n497 = local read "型号"() -> (w1066:string)
                n498 = call <vilib>:"Open Config Data.vi"("configuration file path"=w1071) -> ("refnum"=w1072:T7)  [unwired: 8 in, 2 out]
                n499 = call <vilib>:"Write Key (U32).vi"("section"=w1066, "value"=u32 0, "key"="良品数", "refnum"=w1072) -> ("refnum out"=w1067:T7)  [unwired: 5 in, 2 out]
                n500 = call <vilib>:"Write Key (U32).vi"("section"=w1066, "value"=u32 0, "key"="不良品数", "refnum"=w1067) -> ("refnum out"=w1068:T7)  [unwired: 5 in, 2 out]
                n501 = call <vilib>:"Close Config Data.vi"("refnum"=w1068) -> ()  [unwired: 9 in, 2 out]
              }
            }
            n502 = call "CheckAndControlStateMachine.vi"("Send?"=TRUE, "Mode"=MachineState."Stop") -> ("error out"=w1057:errorcluster)  [unwired: 6 in, 3 out]
            n503 = call <vilib>:"Clear Errors.vi"("error in (no error)"=w1057) -> ("error out"=w1056:errorcluster)  [unwired: 5 in, 1 out]
            n504 = call "CheckAndControlStateMachine.vi"("Mode"=MachineState."Reset", "error in (no error)"=w1056) -> ()  [unwired: 6 in, 4 out]
          }
          event "设置": Value Change {
            n505 = event-data() -> ()  [unwired: 1 in, 1 out]
            n506 = global read "global.vi" "AppPath"() -> (w1076:path)
            n507 = call "2LevelPassword.vi"("路径"=w1076) -> ("Result"=w1075:i32)  [unwired: 10 in]
            n508 = case shown="0.." w1075 {
              selector: w1075 -> [_ w1081]
              tunnel: w1077 -> [_ w1080]
              frame -1, Default {
              }
              frame 0.. {
                n509 = property on="型号" class="CmbBox"() -> ("Strings[]"=w1083:string[], "Value"=w1082:string)  [unwired: 2 in, 2 out]
                n510 = call "setting.vi"("Level"=w1081, "型号"=w1082, "型号表"=w1083) -> ("型号out"=w1078:string, "型号表 out"=w1084:string[])  [unwired: 7 in]
                n511 = property on="型号" class="CmbBox"("Strings[]"=w1084, "Val(Sgnl)"=w1078) -> (error out=w1079:errorcluster)  [unwired: 2 in, 1 out]
                n512 = flat-sequence {
                  tunnel: w1080 -> [w1086]
                  tunnel: w1079 -> [_]
                  frame #0 {
                    n513 = global read "global.vi" "language"() -> (w1085:string)
                    n514 = Generate User Event(user event=w1086, event data cluster=w1085) -> ()  [unwired: 2 in, 2 out]
                  }
                }
              }
            }
          }
          event User Event {
            n515 = event-data() -> ("表格"=w1090:string)  [unwired: 1 in]
            n516 = Spreadsheet String To Array(delimiter (Tab)="\n", format string="%s" ("格式字符串"), spreadsheet string=w1090, array type (2D Dbl)=string[] []) -> (array=w1089:string[])
            n517 = for {
              tunnel: w1089 -> [w1099] mode=indexing
              n518 = Scan From String(format string="%d,%d,%d,%d,%[^,\\r]" ("格式字符串"), input string=w1099) -> (error out=w1092:errorcluster, output 1=w1097:i32, output 2=w1096:i32, output 3=w1095:i32, output 4=w1094:i32, output 5=w1093:string)  [unwired: 7 in, 2 out]
              n519 = case shown="No Error" w1092 {
                tunnel: w1097 -> [w1104 _]
                tunnel: w1096 -> [w1103 _]
                tunnel: w1095 -> [w1102 _]
                tunnel: w1094 -> [w1101 _]
                tunnel: w1093 -> [w1100 _]
                frame No Error {
                  n520 = call "updateTable2.vi"("颜色盒"=w1101, "类型"=w1102, "Value"=w1100, "Row"=w1103, "Col"=w1104) -> ()  [unwired: 6 in, 1 out]
                }
                frame Error {
                }
              }
            }
          }
          event User Event {
            n521 = event-data() -> ("语言"=w1114:string)  [unwired: 1 in]
            n522 = global read "global.vi" "Para"() -> (w1105:T8)
            n523 = case shown="\"EN\"" w1114 {
              tunnel: [w1122 w1132] -> w1113
              tunnel: [1 ("禁用的索引 (列)") 2 ("禁用的索引 (列)")] -> w1110
              tunnel: [u32 20 ("标题.字体:字号") u32 20 ("标题.字体:字号")] -> w1109
              tunnel: ["Nailer打钉功能测试" "Nailer Tester"] -> w1112
              tunnel: ["时间(秒)" ("X标尺.名称标签.文本") "Time(S)" ("X标尺.名称标签.文本")] -> w1107
              tunnel: ["幅值(安培)" ("X标尺.名称标签.文本") "Current Level(A)" ("X标尺.名称标签.文本")] -> w1106
              tunnel: w1105 -> [w1116 w1126]
              frame "CN", Default {
                n524 = Unbundle By Name(w1116) -> ("CurrentType"=w1115:enum16{"RMS均方根值", "AVG平均值"})
                n525 = case shown="\"AVG平均值\"" w1115 {
                  tunnel: [string[] ["项目\nItem", "时间\nTime", "最大电流(A)\nPeak amps", "均方根电流(A)\nRMS amps", "能量\nPower", "打钉时间(ms)\nRetraction time", "结果\nResult"] ("行首字符串[]") string[] ["项目\nItem", "时间\nTime", "最大电流(A)\nPeak amps", "平均电流(A)\nAVG amps", "能量\nPower", "打钉时间(ms)\nRetraction time", "结果\nResult"] ("行首字符串[]")] -> w1122
                  frame "RMS均方根值", Default {
                  }
                  frame "AVG平均值" {
                  }
                }
              }
              frame "EN" {
                n526 = Unbundle By Name(w1126) -> ("CurrentType"=w1125:enum16{"RMS均方根值", "AVG平均值"})
                n527 = case shown="\"RMS均方根值\", Default" w1125 {
                  tunnel: [string[] ["TestItem", "DateTime", "Max Current(A)", "RMS Current(A)", "Power", "Time(ms)", "Result"] ("行首字符串[]") string[] ["TestItem", "DateTime", "Max Current(A)", "AVG Current(A)", "Power", "Time(ms)", "Result"] ("行首字符串[]")] -> w1132
                  frame "RMS均方根值", Default {
                  }
                  frame "AVG平均值" {
                  }
                }
              }
            }
            n528 = local write "标题"(w1112) -> ()
            n529 = property on="项目" class="Tbl (strict)"("Column Headers[]"=w1113) -> ()  [unwired: 2 in, 2 out]
            n530 = property on="波形图" class="WFGraph (strict)"("XScale.NameLbl.Text"=w1107, "YScale.NameLbl.Text"=w1106) -> ()  [unwired: 2 in, 2 out]
            n531 = property class="VI"() -> ("Panel"=w1111:refnum<vi>)  [unwired: 2 in, 2 out]
            n532 = call "控件文本.vi"("数组"=string[][] [["型号", "型号", "Model"], ["设置", "设置", "Setting"], ["Exit", "退出", "Exit"], ["清零", "清零", "Reset"], ["开始", "开始", "Start"], ["Stop", "停止", "Stop"], ["PLC连接状态", "PLC连接状态", "PLC Connection State"]], "字号"=w1109, "选择列"=w1110, "引用"=w1111) -> ()  [unwired: 8 in]
          }
        }
      }
      n533 = while {
        tunnel: [w131] -> w102
        tunnel: [w130] -> w103
        tunnel: w105 -> [w133]
        tunnel: w104 -> [w132]
        stop <- FALSE stop-if-true
        n534 = local read "FirstTime"() -> (w129:bool)
        n535 = case shown="False" w129 {
          tunnel: w133 -> [w137 w215]
          tunnel: w132 -> [w138 w214]
          tunnel: [w136 w213] -> w131
          tunnel: [w135 w212] -> w130
          frame True {
            n536 = flat-sequence {
              tunnel: w138 -> [w144]
              tunnel: w137 -> [w143]
              tunnel: [w142] -> w140
              tunnel: [w141] -> w139
              tunnel: [w172] -> w135
              tunnel: [w173] -> w136
              tunnel: w140 -> [w173]
              tunnel: w139 -> [w172]
              frame #0 {
                n537 = global read "global.vi" "High Volt alarm (0.01V)"() -> (w148:string)
                n538 = global read "global.vi" "Low Volt alarm (0.01V)"() -> (w147:string)
                n539 = To Unsigned Word Integer(number=0) -> (unsigned 16bit integer=w165:u16)
                n540 = Decimal String To Number(string=w148, default (0L)=w165) -> (number=w164:u16)  [unwired: 1 in, 1 out]
                n541 = To Unsigned Word Integer(number=0) -> (unsigned 16bit integer=w163:u16)
                n542 = Decimal String To Number(string=w147, default (0L)=w163) -> (number=w161:u16)  [unwired: 1 in, 1 out]
                n543 = global read "global.vi" "Modbus RTU Address"() -> (w146:string)
                n544 = call-dynamic "Write Single Holding Register.vi"("error in"=w143, "register to write"=w164, "address"=u16 0, "Modbus master in"=w144) -> ("error out"=w169:errorcluster, "Modbus master out"=w170:refnum<class "Modbus Master.lvclass">)  [unwired: 6 in]
                n545 = call-dynamic "Write Single Holding Register.vi"("error in"=w169, "register to write"=w161, "address"=u16 1, "Modbus master in"=w170) -> ("error out"=w159:errorcluster, "Modbus master out"=w158:refnum<class "Modbus Master.lvclass">)  [unwired: 6 in]
                n546 = To Unsigned Word Integer(number=0) -> (unsigned 16bit integer=w156:u16)
                n547 = Decimal String To Number(string=w146, default (0L)=w156) -> (number=w155:u16)  [unwired: 1 in, 1 out]
                n548 = global read "global.vi" "Currrent Range"() -> (w145:string)
                n549 = call-dynamic "Write Single Holding Register.vi"("error in"=w159, "register to write"=w155, "address"=u16 2, "Modbus master in"=w158) -> ("error out"=w154:errorcluster, "Modbus master out"=w153:refnum<class "Modbus Master.lvclass">)  [unwired: 6 in]
                n550 = To Unsigned Word Integer(number=0) -> (unsigned 16bit integer=w152:u16)
                n551 = Decimal String To Number(string=w145, default (0L)=w152) -> (number=w149:u16)  [unwired: 1 in, 1 out]
                n552 = call-dynamic "Write Single Holding Register.vi"("error in"=w154, "register to write"=w149, "address"=u16 3, "Modbus master in"=w153) -> ("error out"=w141:errorcluster, "Modbus master out"=w142:refnum<class "Modbus Master.lvclass">)  [unwired: 6 in]
              }
              frame #1 {
                n553 = local write "FirstTime"(FALSE ("FirstTime")) -> ()
              }
            }
          }
          frame False {
            n554 = control-ref of="This VI"() -> (w218:refnum<vi>)
            n555 = Open VI Reference(type specifier VI Refnum (for type only)=w218, vi path=path "C:/Users/trila/Desktop/NailerTesterCode_ApplyTrace/NailerTesterCode/Alarm_Battery.vi") -> (vi reference=w216:refnum<vi>)  [unwired: 4 in, 1 out]
            n556 = call-dynamic "Read Input Registers.vi"("error in"=w215, "number of inputs"=u16 8, "starting address"=u16 0, "Modbus master in"=w214) -> ("error out"=w212:errorcluster, "register values"=w219:u16[], "Modbus master out"=w213:refnum<class "Modbus Master.lvclass">)  [unwired: 5 in]
            "register data" <- w219
            n557 = Index Array(array=w219, index=1) -> (element=w205:u16)
            n558 = Index Array(array=w219, index=0) -> (element=w201:u16)
            n559 = Index Array(array=w219, index #1=4 ("index"), index #2=5 ("index")) -> (element #1=w195:u16, element #2=w194:u16)
            n560 = Index Array(array=w219, index #1=2 ("index"), index #2=3 ("index")) -> (element #1=w196:u16, element #2=w197:u16)
            n561 = Index Array(array=w219, index=6) -> (element=w211:u16)
            n562 = Index Array(array=w219, index=7) -> (element=w207:u16)
            n563 = To Double Precision Float(number=w205) -> (double precision float=w204:dbl)
            n564 = To Double Precision Float(number=w201) -> (double precision float=w202:dbl)
            n565 = Number To Hexadecimal String(2:w211) -> (0:w210:string)  [unwired: 1 in]
            n566 = Number To Hexadecimal String(2:w207) -> (0:w208:string)  [unwired: 1 in]
            n567 = Multiply(x=0.01, y=w204) -> (x*y=→"Current(A)":dbl)
            n568 = Insert Into Array(array=dbl[] [], new element #1=w195, new element #2=w194) -> (w193:dbl[])  [unwired: 1 in]
            n569 = Multiply(x=0.01, y=w202) -> (x*y=→"Battery Voltage":dbl)
            n570 = Insert Into Array(array=dbl[] [], new element #1=w196, new element #2=w197) -> (w198:dbl[])  [unwired: 1 in]
            n571 = Equal?(x=w210, y="FFFF") -> (x = y?=→"HighAlarm":bool)
            n572 = Equal?(x=w208, y="FFFF") -> (x = y?=w174:bool)
            "Battery Low Voltage" <- w174
            n573 = Type Cast(type=0.0, x=w193) -> (*(type *) &x=→"Energy(Wh)":dbl)
            n574 = Type Cast(type=0.0, x=w198) -> (*(type *) &x=w199:dbl)
            n575 = Multiply(x=w199, y=0.1) -> (x*y=→"Power(W)":dbl)
            n576 = case shown="True" w174 {
              tunnel: w216 -> [w222 w229]
              frame False {
                n577 = flat-sequence {
                  tunnel: w222 -> [w224]
                  frame #0 {
                    n578 = local read "isOpen"() -> (w223:bool)
                    n579 = case shown="True" w223 {
                      tunnel: w224 -> [_ w227]
                      frame False {
                      }
                      frame True {
                        n580 = invoke class="VI" method="Abort VI"(reference=w227) -> (reference out=w226:refnum<vi>, error out=w225:errorcluster)  [unwired: 2 in, 1 out]
                        n581 = invoke class="VI" method="FP.Close"(reference=w226, error in=w225) -> ()  [unwired: 1 in, 3 out]
                      }
                    }
                  }
                  frame #1 {
                    n582 = local write "isOpen"(FALSE) -> ()
                  }
                }
              }
              frame True {
                n583 = flat-sequence {
                  tunnel: w229 -> [w231]
                  frame #0 {
                    n584 = local read "isOpen"() -> (w230:bool)
                    n585 = case shown="False" w230 {
                      tunnel: w231 -> [_ w236]
                      frame True {
                      }
                      frame False {
                        n586 = invoke class="VI" method="FP.Open"(reference=w236, "Activate"=TRUE ("Activate?"), "State"=T3."Standard") -> (reference out=w235:refnum<vi>, error out=w234:errorcluster)  [unwired: 2 in, 3 out]
                        n587 = invoke class="VI" method="Run VI"(reference=w235, error in=w234, "Wait until done"=FALSE ("Wait Until Done"), "Auto Dispose Ref"=TRUE ("Auto Dispose Reference")) -> ()  [unwired: 1 in, 5 out]
                      }
                    }
                  }
                  frame #1 {
                    n588 = local write "isOpen"(TRUE) -> ()
                  }
                }
              }
            }
          }
        }
      }
      n589 = call "HostConnectionSubloop.vi"("error in (no error)"=w111) -> ()  [unwired: 10 in, 1 out]
      n590 = call-dynamic "Shutdown.vi"("error in"=w103, "Modbus master in"=w102) -> ()  [unwired: 9 in, 1 out]
    }
  }
